vi "VIH UI - Property Page - Group Rule.vi"() -> ()   [LabVIEW 2014]
doc: "::: VI Helpeks :::\nCopyright (c) 2000-2026 Konstantin Shifershteyn. All rights reserved."
uses:
  _VIH HelpGen.llb/VIH HelpGen Typedef - Enum - Description Mode.ctl
  _VIH HelpGen.llb/VIH HelpGen Typedef - Enum - Default,Enable,Disable.ctl
  _VIH UI Controls.llb/VIH UI Control - Button - Insert HREF.ctl
  _VIH UI Controls.llb/VIH UI Control - Button - Insert Bold.ctl
  _VIH UI Controls.llb/VIH UI Control - Button - Insert Italic.ctl
  _VIH UI Controls.llb/VIH UI Control - Button - Insert Underline.ctl
  _VIH Project Manager.llb/VIH Project Tree Typedef - Tree Refnum.ctl
  VIH UI Typedef - Property Page ExtCommand.ctl
  <vilib>/Utility/miscctls.llb/LVPositionTypeDef.ctl
  <vilib>/Utility/miscctls.llb/LVPointTypeDef.ctl
  <vilib>/Utility/miscctls.llb/LVRowAndColumnUnsignedTypeDef.ctl
  <vilib>/Utility/miscctls.llb/LVSelectionTypeDef.ctl
  _VIH Support Library.llb/VIH Utility - APP - Is Value Changed (STR).vi
panel:
  out "CategoryTitle":string
  in  "%UPDATE":bool
  in  "%STOP":bool
  in  "Category List":i32(listbox)
  in  "TreeRef":T1
  in  "Tab Control":enum32{"0", "1", "2", "3", "4", "5", "6", "7"}(tab) caption="Group Rule"
  out "PI_AddInfo":string caption="Additional Information"
  out "PI_Email":string caption="Contact E-mail"
  out "PI_Website":string caption="Website"
  out "PI_Version":string caption="Version"
  out "PI_Copyright":string caption="Legal Copyright"
  out "PI_Company":string caption="Company Name"
  out "PI_Author":string caption="Author Name"
  out "PI_Product":string caption="Product Name"
  in  "ProductInfoText":string caption="Product Info section"
  in  "ProductInfoMode":u16(ring) caption="Product Info mode" items=["Default", "Custom", "Disable"]
  in  "BuildHelp":T2 caption="Build help for files of this group"
  in  "Group Name":string
  in  "Comments":string
  in  "Custom_JS Dir":i16(ring) caption="Default/Custom selector" items=["Default", "Custom"]
  in  "Dst_JS Dir":path caption="Subfolder to save JavaScript files"
  in  "Custom_CSS Dir":i16(ring) caption="Default/Custom selector" items=["Default", "Custom"]
  in  "Dst_CSS Dir":path caption="Subfolder to save CSS files"
  in  "Custom_Image Dir":i16(ring) caption="Default/Custom selector" items=["Default", "Custom"]
  in  "Dst_Image Dir":path caption="Subfolder to save image files"
  in  "Custom_HTML Dir":i16(ring) caption="Default/Custom selector" items=["Default", "Custom"]
  in  "Dst_HTML Dir":path caption="Subfolder to save HTML files"
  out "Build Root Dir":path caption="Build Root Folder"
  in  "Src_VI Template":path caption="VI Help Template File"
  in  "Custom_VI Template":i16(ring) caption="Default/Custom selector" items=["Default", "Custom"]
  in  "Src_Menu Template":path caption="Menu Help Template File"
  in  "Custom_Menu Template":i16(ring) caption="Default/Custom selector" items=["Default", "Custom"]
  in  "Src_PolyVI Template":path caption="Polymorphic VI Help Template File"
  in  "Custom_PolyVI Template":i16(ring) caption="Default/Custom selector" items=["Default", "Custom"]
  out "JS File":path caption="JS File Path"
  in  "JS List":i32[](listbox) caption="JavaScript Files"
  in  "%JS List_Add":bool caption="Add JavaScript File"
  in  "%JS List_Remove":bool caption="Remove JavaScript File"
  in  "Override_JS Files":bool caption="Override default JS file set"
  out "CSS File":path caption="CSS File Path"
  in  "CSS List":i32[](listbox) caption="CSS Files"
  in  "%CSS List_Add":bool caption="Add CSS File"
  in  "%CSS List_Remove":bool caption="Remove CSS File"
  in  "Override_CSS Files":bool caption="Override default CSS file set"
  in  "VIDetailsMode":T3 caption="Default VI details mode"
  in  "PVIIDscrMode":T3 caption="Default Polymorphic VI Instance description mode"
  in  "MenuItemIcons":T2 caption="Generate Palette Item Icons"
  in  "MenuDscrMode":T3 caption="Default Palette description mode"
  in  "VIDscrMode":T3 caption="Default VI description mode"
  in  "Ctl_EnumValues":T2 caption="Build list of Enum and Ring values"
  in  "Ctl_ClustMembers":T2 caption="Expand cluster members"
  in  "Ctl_DscrMode":T3 caption="VI Controls/Terminals description mode"
  in  "%CtrlRule_Insert_<I>":T4 caption="Format as Italic"
  in  "%CtrlRule_Insert_<U>":T5 caption="Format as Underline"
  in  "%CtrlRule_Insert_<B>":T6 caption="Format as Bold"
  in  "%CtrlRule_Insert_HREF":T7 caption="Insert Reference"
  in  "CtrlRule_Description":string caption="Description"
  in  "CtrlRule_CustomName":string caption="Custom Control Name"
  in  "CtrlRule_DscrMode":T3 caption="Description mode"
  in  "CtrlRule_CustomRule":bool caption="Enable custom rule"
  in  "CtrlRule_CtrlID":string caption="Control Identifier"
  in  "%CtrlRule_Edit_Enum":bool caption="Edit Enumerated Values Description"
  in  "CtrlRule_EnumValues":T2 caption="Enum and Ring values"
  in  "CtrlRule_ClustMembers":T2 caption="Cluster members"
  in  "%CtrlRule_Copy":bool caption="Copy"
  in  "%CtrlRule_Paste":bool caption="Paste"
  in  "%CtrlRule_Import":bool caption="Import VI Terminal Controls"
  in  "CtrlRule List":i32[](listbox) caption="Control List"
  in  "%CtrlRule_Remove":bool caption="Remove"
  in  "%CtrlRule_Add":bool caption="Add"
  in  "Override_Ctl Rules":bool caption="Override default Control Rules definition"
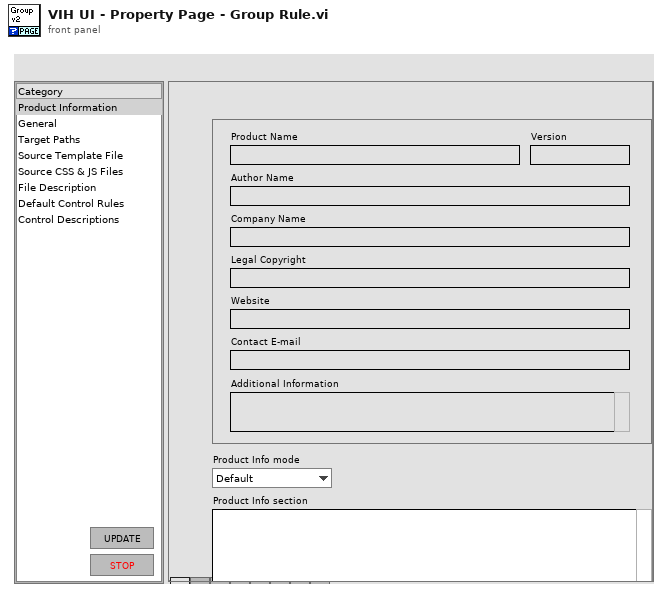
[diagram p1: front panel]
types:
  T1 = typedef "VIH Project Tree Typedef - Tree Refnum.ctl" = refnum<vi>
  T2 = typedef "VIH HelpGen Typedef - Enum - Default,Enable,Disable.ctl" = enum16{"Default", "Enable", "Disable"}
  T3 = typedef "VIH HelpGen Typedef - Enum - Description Mode.ctl" = enum16{"Default", "Description", "Description1", "Description2", "Custom", "None"}
  T4 = typedef "VIH UI Control - Button - Insert Italic.ctl" = bool
  T5 = typedef "VIH UI Control - Button - Insert Underline.ctl" = bool
  T6 = typedef "VIH UI Control - Button - Insert Bold.ctl" = bool
  T7 = typedef "VIH UI Control - Button - Insert HREF.ctl" = bool
  T8 = typedef "VIH UI Typedef - Property Page ExtCommand.ctl" = cluster{"Action":string, "Project Tree":T1, "Params":string[]}
  T9 = enum16{"Open", "Close", "Update", "Set Category"}
  T10 = enum32{"Invalid", "Standard", "Closed", "Hidden", "Minimized", "Maximized"}
  T11 = enum8{"Enabled", "Disabled", "Disabled and Grayed Out"}
  T12 = typedef "LVSelectionTypeDef.ctl" = cluster{"Selection Start":u32, "Selection End":u32}
  T13 = enum16{"get", "get all", "set", "Init", "delete"}
  T14 = typedef "eventvkey.ctl" = enum16{"ASCII", "Enter", "Return", "Shift", "Ctrl", "Alt", "Cmd", "Opt", "Caps", "NumLock", "Clear", "Break", "Up", "Down", "Left", "Right", "Insert", "Delete", "Home", "End", "PageUp", "PageDown", "Escape", "Help", "Pause", "ScrollLock", "F1", "F2", "F3", "F4", "F5", "F6", "F7", "F8", "F9", "F10", "F11", "F12", "F13", "F14", "F15", "F16", "F17", "F18", "F19", "F20", "F21", "F22", "F23", "F24", "Play", "VolumeUp", "VolumeDown", "Mute", "Two Byte Char"}
  T15 = cluster{"Shift":bool, "Ctrl":bool, "Alt":bool, "Cmd":bool, "Opt":bool}
  T16 = typedef "VIH HelpGen Typedef - Cluster - Group Rule.ctl" = cluster{"Source Root Dir":path, "Build Root Dir":path, "BuildHelp":T2, "Source Paths":T17, "Target Paths":T18, "VIDscrMode":T3, "MenuDscrMode":T3, "MenuItemIcons":T2, "Control Rules":T19[], "Flags":T21, "Ctl_DscrMode":T3, "Ctl_ClustMembers":T2, "Ctl_EnumValues":T2, "%Comments":string, "PVIIDscrMode":T3, "VIDetailsMode":T3, "ProductInfoMode":T2, "ProductInfoText":string}
  T17 = typedef "VIH HelpGen Typedef - Cluster - Group Rule - Source Paths.ctl" = cluster{"CSS Files":path[], "JS Files":path[], "VI Template":path, "Menu Template":path, "PolyVI Template":path}
  T18 = typedef "VIH HelpGen Typedef - Cluster - Group Rule - Target Paths.ctl" = cluster{"HTML Dir":path, "Image Dir":path, "CSS Dir":path, "JS Dir":path}
  T19 = typedef "VIH HelpGen Typedef - Cluster - Control Rule.ctl" = cluster{"CtrlID":string, "CustomRule":bool, "DscrMode":T3, "Description":string, "ClusterMembers":T2, "EnumValues":T2, "EnumValDscr":T20[], "CustomName":string}
  T20 = typedef "VIH HelpGen Typedef - Cluster - Enum Value Info.ctl" = cluster{"Value":ext, "String":string, "Description":string}
  T21 = typedef "VIH HelpGen Typedef - Cluster - Group Rule - Flags.ctl" = cluster{"Override CSS Files":bool, "Override JS Files":bool, "Override Ctl Rules":bool}
  T22 = typedef "LVPoint32TypeDef.ctl" = cluster{"Horizontal":i32, "Vertical":i32}
  T23 = typedef "LVRowAndColumnTypeDef.ctl" = cluster{"Row":i32, "Column":i32}
  T24 = typedef "lveventtype.ctl" = enum32{"Null", "Timeout", "Annotation Menu Selection", "Annotation Menu Selection?", "App Instance Close", "App Instance Close?", "Autoscale Range Change", "Bookmark Info Change", "Cell Edit", "Cell Edit?", "Cursor Grab", "Cursor Grab?", "Cursor Menu Selection", "Cursor Menu Selection?", "Cursor Move", "Cursor Release", "Data Change", "Direction Change", "Display State Change", "Drag Ended", "Drag Enter", "Drag Leave", "Drag Over", "Drag Source Update", "Drag Starting", "Drag Starting?", "Drop", "Exec State Change", "Key Down", "Key Down?", "Key Repeat", "Key Repeat?", "Key Up", "Listbox Double Click", "Menu Activation?", "Menu Selection (App)", "Menu Selection? (App)", "Menu Selection (User)", "Mouse Down", "Mouse Down?", "Mouse Enter", "Mouse Leave", "Mouse Move", "Mouse Up", "Mouse Wheel", "NI Security User Change (App)", "Pane Size", "Panel Close", "Panel Close?", "Panel Resize", "Plot Attribute Change", "Scale Range Change", "Shortcut Menu Activation?", "Shortcut Menu Selection (App)", "Shortcut Menu Selection? (App)", "Shortcut Menu Selection (User)", "Tree Double Click", "Tree Drag", "Tree Drag?", "Tree Drop", "Tree Drop?", "Tree Item Close", "Tree Item Close?", "Tree Item Open", "Tree Item Open?", "User Event", "Value Change"}
  T25 = typedef "LVPointTypeDef.ctl" = cluster{"Horizontal":i16, "Vertical":i16}
  T26 = typedef "LVPositionTypeDef.ctl" = cluster{"Left":i32, "Top":i32}
  T27 = typedef "LVRowAndColumnUnsignedTypeDef.ctl" = cluster{"Row":u32, "Column":u32}
  T28 = cluster{"Array out":string[], "Group Rule out":T16}
  T29 = typedef "VIH HelpGen Typedef - Product Info Cluster.ctl" = cluster{"ProductName":string, "Version":string, "Author":string, "Company":string, "Copyright":string, "Website":string, "Email":string, "AddInfo":string}
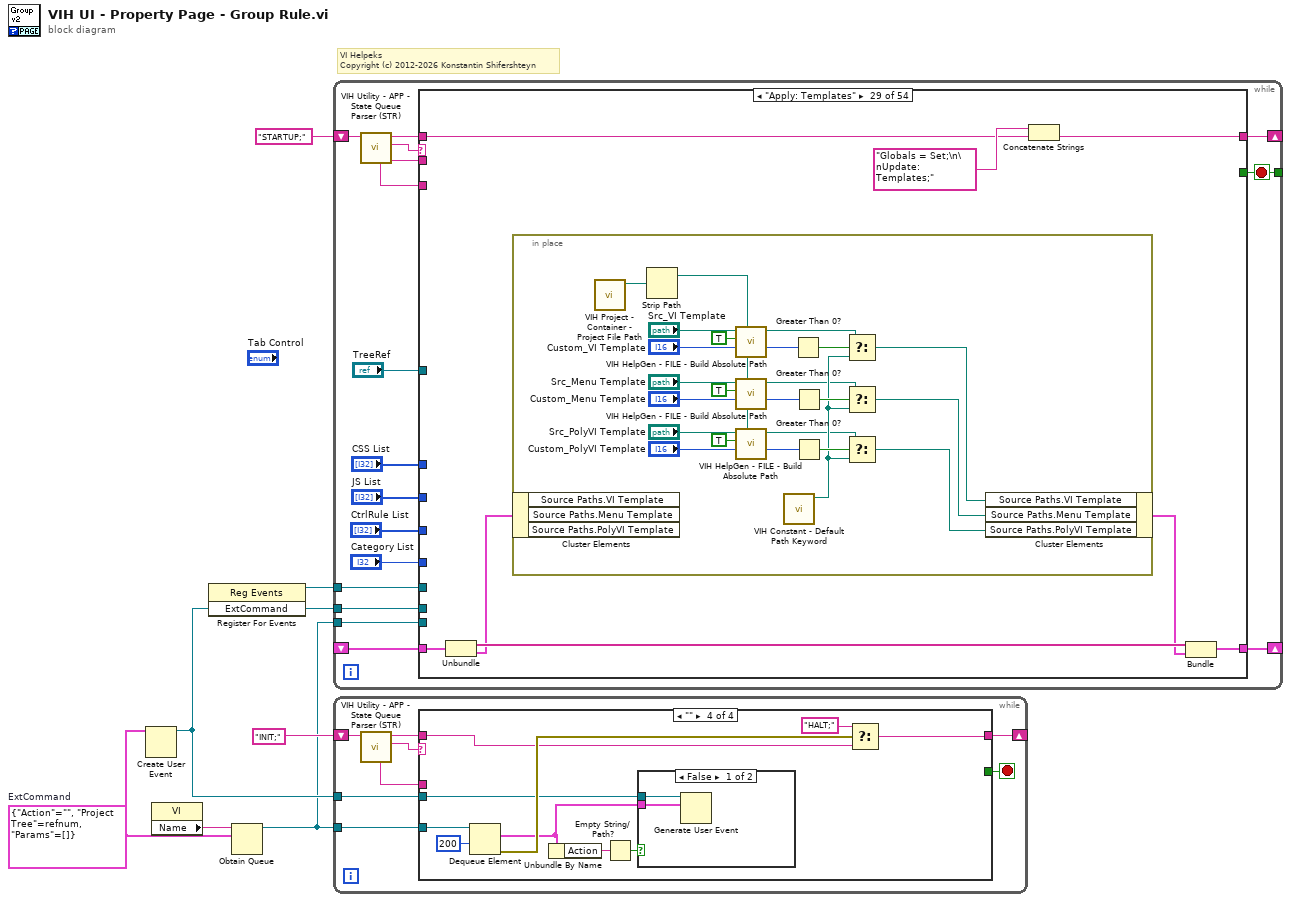
[diagram p0: block diagram]
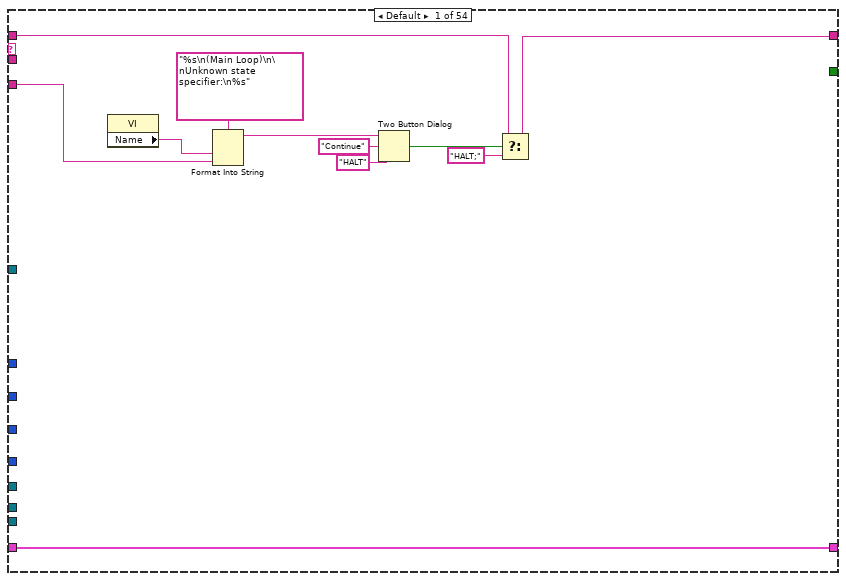
[diagram p2: hidden frame]
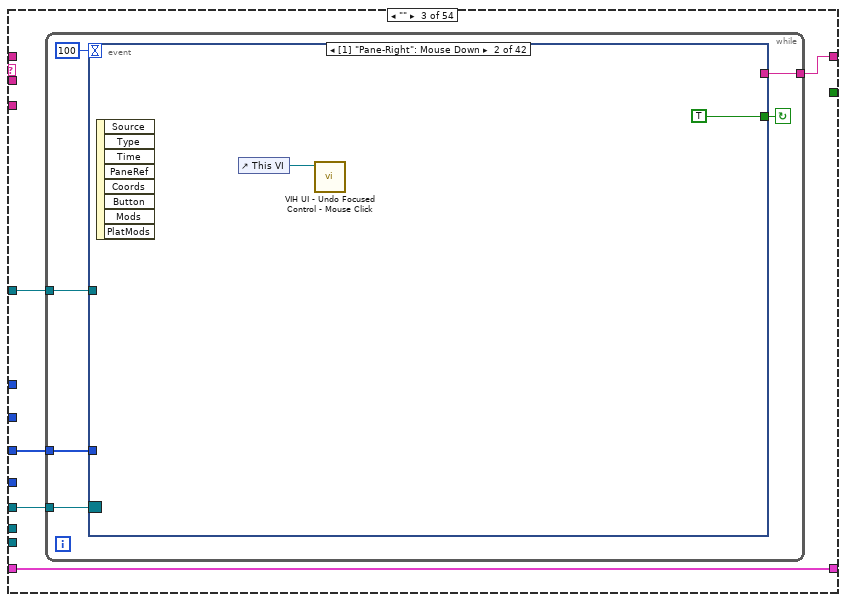
[diagram p4: hidden frame]
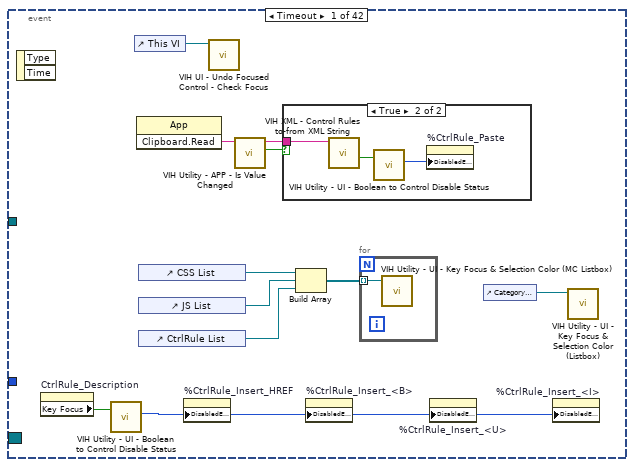
[diagram p5: hidden frame]
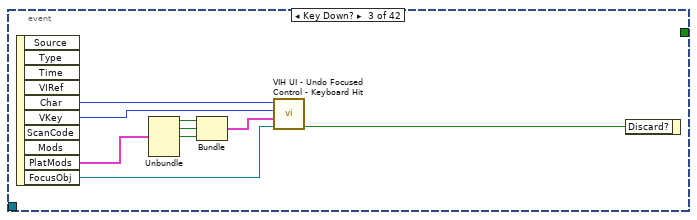
[diagram p7: hidden frame]
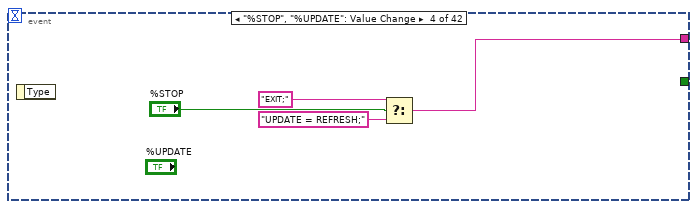
[diagram p8: hidden frame]
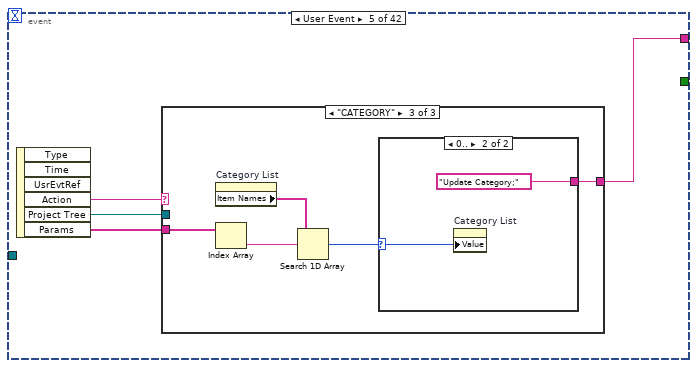
[diagram p9: hidden frame]
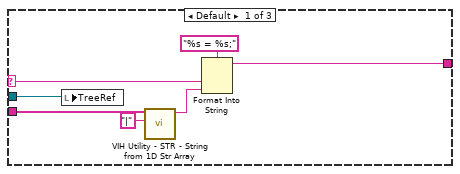
[diagram p10: hidden frame]
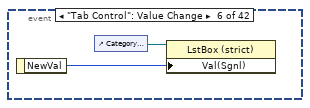
[diagram p13: hidden frame]
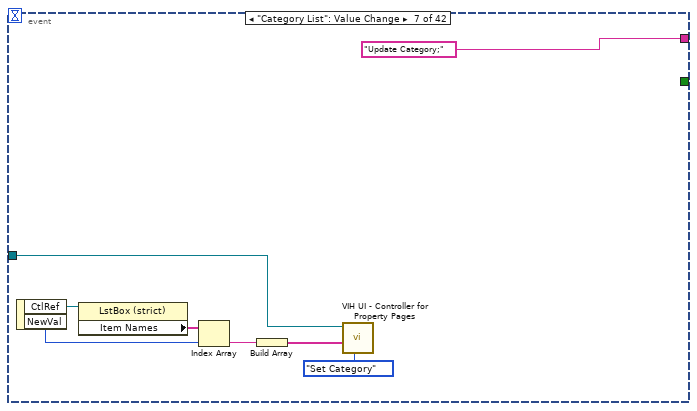
[diagram p14: hidden frame]
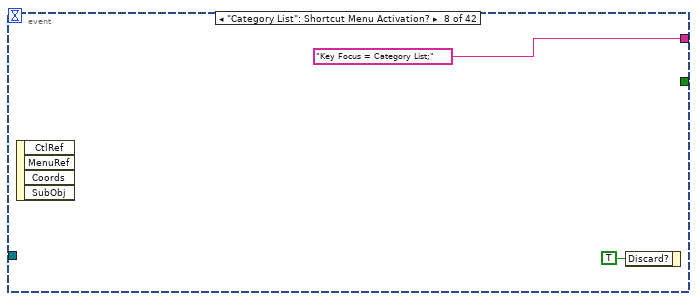
[diagram p15: hidden frame]
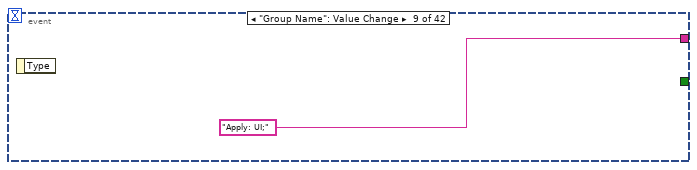
[diagram p16: hidden frame]
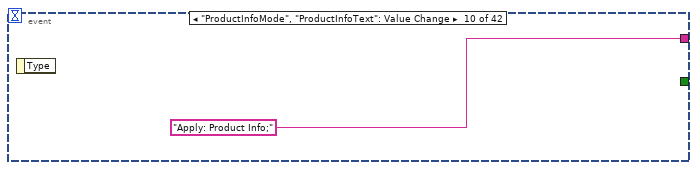
[diagram p17: hidden frame]
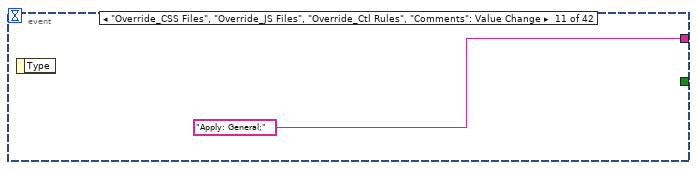
[diagram p18: hidden frame]
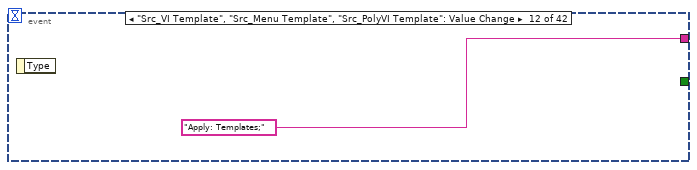
[diagram p19: hidden frame]
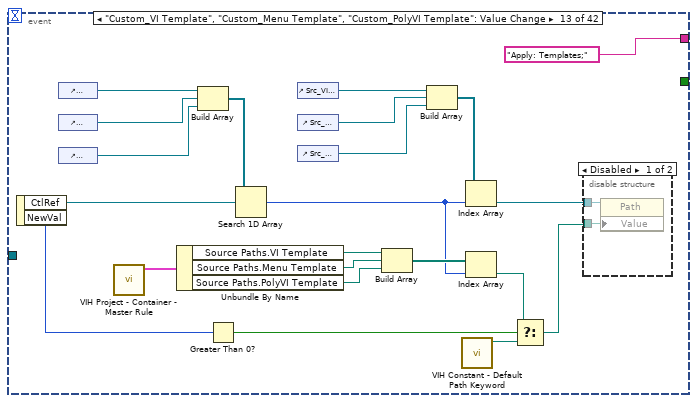
[diagram p20: hidden frame]
diagram:
  w1 = T8 {"Action"="", "Project Tree"=refnum, "Params"=[]}  # ExtCommand
  # "VI Helpeks\nCopyright (c) 2012-2026 Konstantin Shifershteyn"
  n1 = Create User Event(user event datatype=w1) -> (user event=w3:refnum<user-event>)  [unwired: 1 in, 1 out]
  n2 = property class="VI"() -> ("Name"=w6:string)  [unwired: 2 in, 2 out]
  n3 = register-events(w3) -> (reference out=w5:refnum<event-registration>)  [unwired: 2 in, 1 out]
  n4 = Obtain Queue(name (unnamed)=w6, element data type=w1) -> (queue out=w2:refnum<queue>)  [unwired: 3 in, 2 out]
  n5 = while {
    shift-right: [w21] -> _
    shift-left: "STARTUP;" -> [w24]
    tunnel: [w19] -> _
    tunnel: w5 -> [w18]
    tunnel: w3 -> [w17]
    tunnel: w2 -> [w16]
    shift-right: [w13] -> _
    shift-left: _ -> [w12]
    stop <- w19 stop-if-true
    n6 = call "VIH Utility - APP - State Queue Parser (STR).vi"("input queue"=w24) -> ("state parameters"=w15:string, "state"=w23:string, "remained queue"=w20:string, "complete state specifier"=w22:string)  [unwired: 5 in]
    n7 = case shown="\"Apply: Templates\"" w23 {
      tunnel: w22 -> [w31 _ _ _ _ _ _ _ _ w438 _ _ _ _ _ _ _ _ _ _ _ _ _ _ _ _ _ _ _ _ _ _ _ _ _ _ _ _ _ _ _ _ _ _ _ _ _ _ _ _ _ _ _ _]
      tunnel: [w26 w36 w41 "INIT;\nUPDATE;" w383 "HALT;" w411 w414 w430 w440 w463 w466 w470 w486 w493 w510 w519 w563 w602 w636 w663 w682 w697 w715 w726 w727 w740 w753 w778 w807 w824 w842 w872 w899 w948 w955 w979 w995 w1031 w1051 w1075 w1084 w1093 w1105 w1131 w1155 w1170 w1179 w1188 w1200 w1226 w1250 w1265 w1267] -> w21
      tunnel: w20 -> [w27 w36 _ _ w383 _ w411 w414 w431 w440 w463 w466 w470 w486 w493 w510 w519 w563 w602 w636 w663 w682 w697 w715 w726 w728 w746 w754 w779 w808 w824 w842 w877 w901 w948 w960 w984 w1002 w1036 w1058 w1075 w1084 w1093 w1109 w1136 w1160 w1170 w1179 w1188 w1204 w1231 w1255 w1265 w1267]
      tunnel: [_ _ _ _ _ _ TRUE _ _ _ _ _ _ _ _ _ _ _ _ _ _ _ _ _ _ _ _ _ _ _ _ _ _ _ _ _ _ _ _ _ _ _ _ _ _ _ _ _ _ _ _ _ _ _] -> w19
      tunnel: w18 -> [_ _ w42 _ _ _ w410 _ _ _ _ _ _ _ _ _ _ _ _ _ _ _ _ _ _ _ _ _ _ _ _ _ _ _ _ _ _ _ _ _ _ _ _ _ _ _ _ _ _ _ _ _ _ _]
      tunnel: w17 -> [_ _ _ _ _ _ w409 _ _ _ _ _ _ _ _ _ _ _ _ _ _ _ _ _ _ _ _ _ _ _ _ _ _ _ _ _ _ _ _ _ _ _ _ _ _ _ _ _ _ _ _ _ _ _]
      tunnel: w16 -> [_ _ _ _ _ _ w407 _ _ _ _ _ _ _ _ _ _ _ _ _ _ _ _ _ _ _ _ _ _ _ _ _ _ _ _ _ _ _ _ _ _ _ _ _ _ _ _ _ _ _ _ _ _ _]
      tunnel: w15 -> [_ _ _ _ _ _ _ _ w418 w439 _ w464 w468 _ _ _ _ _ _ w625 w654 _ w684 _ _ _ _ _ _ _ _ w825 _ w894 _ _ _ w993 w1020 w1049 _ _ _ _ _ _ _ _ _ _ _ _ _ _]
      tunnel: "Category List" -> [_ _ _ _ _ _ _ _ _ _ w460 _ _ _ _ _ _ _ _ _ _ _ _ _ _ _ _ _ _ _ _ _ _ _ _ _ _ _ _ _ _ _ _ _ _ _ _ _ _ _ _ _ _ _]
      tunnel: [w25 w37 w40 w348 w382 w392 w405 w413 w428 w442 w459 w465 w469 w485 w489 w509 w518 w562 w601 w635 w662 w681 w696 w714 w721 w732 w743 w758 w783 w812 w823 w841 w873 w898 w945 w956 w980 w997 w1032 w1053 w1074 w1081 w1092 w1106 w1132 w1156 w1169 w1176 w1187 w1201 w1227 w1251 w1264 w1266] -> w13
      tunnel: w12 -> [w25 w37 w40 w348 w382 w392 w405 w413 w425 w441 w459 w465 w469 w485 w489 w509 w518 w562 w601 w635 w662 w681 w696 w714 w721 w734 w745 w760 w785 w814 w823 w841 w874 w900 w945 w957 w981 w998 w1033 w1054 w1074 w1081 w1092 w1107 w1133 w1157 w1169 w1176 w1187 w1202 w1228 w1252 w1264 w1266]
      tunnel: "CtrlRule List" -> [_ _ w39 _ _ _ _ _ _ _ _ _ _ _ _ _ _ _ _ _ _ _ w686 _ _ _ _ _ _ _ _ w831 w866 w892 w946 w953 _ _ _ _ _ _ _ _ _ _ _ _ _ _ _ _ _ _]
      tunnel: "CSS List" -> [_ _ _ _ _ _ _ _ _ _ _ _ _ _ _ _ _ _ _ w627 _ _ _ _ _ _ _ _ _ _ _ _ _ _ _ _ _ _ _ _ _ w1078 _ w1097 w1129 _ _ _ _ _ _ _ _ _]
      tunnel: "JS List" -> [_ _ _ _ _ _ _ _ _ _ _ _ _ _ _ _ _ _ _ _ w653 _ _ _ _ _ _ _ _ _ _ _ _ _ _ _ _ _ _ _ _ _ _ _ _ _ _ w1171 _ w1190 w1224 _ _ _]
      tunnel: "TreeRef" -> [_ _ w38 _ _ _ _ _ _ _ _ _ _ _ w490 _ _ w535 w578 _ _ _ _ _ w719 _ _ _ _ _ _ _ _ w890 _ _ _ _ _ w1048 _ _ _ _ _ _ _ _ _ _ _ _ _ _]
      frame Default {
        n8 = property class="VI"() -> ("Name"=w30:string)  [unwired: 2 in, 2 out]
        n9 = Format Into String(format string="%s\n(Main Loop)\n\nUnknown state specifier:\n%s", w30, w31) -> (resulting string=w34:string)  [unwired: 2 in, 1 out]
        n10 = Two Button Dialog(message=w34, 1:"HALT" ("F button name (\"Cancel\")"), 2:"Continue" ("T button name (\"OK\")")) -> (T button?=w28:bool)
        n11 = Select(t=w27, s=w28, f="HALT;") -> (s? t:f=w26:string)
      }
      frame "#" {
      }
      frame "" {
        n12 = while {
          tunnel: w42 -> [w47]
          tunnel: [w46] -> w41
          tunnel: w39 -> [w45]
          tunnel: w38 -> [w44]
          stop <- w43 continue-if-true
          n13 = event shown="[1] \"Pane-Right\": Mouse Down" {
            selector: w47 -> [_ _ _ _ _ _ _ _ _ _ _ _ _ _ _ _ _ _ _ _ _ _ _ _ _ _ _ _ _ _ _ _ _ _ _ _ _ _ _ _ _ _]
            dyn-events: _ -> [_ _ _ _ _ _ _ _ _ _ _ _ _ _ _ _ _ _ _ _ _ _ _ _ _ _ _ _ _ _ _ _ _ _ _ _ _ _ _ _ _ _]
            timeout: 100 -> [_ _ _ _ _ _ _ _ _ _ _ _ _ _ _ _ _ _ _ _ _ _ _ _ _ _ _ _ _ _ _ _ _ _ _ _ _ _ _ _ _ _]
            tunnel: [_ _ _ w76 w82 _ "Update Category;" ("string") "Key Focus = Category List;" ("output string") "Apply: UI;" ("string") "Apply: Product Info;" ("string") "Apply: General;" ("string") "Apply: Templates;" ("string") "Apply: Templates;" ("string") "Apply: Target Paths;" ("string") "Apply: Target Paths;" ("string") "Apply: Item Rules;" ("string") "Apply: Item Rules;" ("string") "CtrlRule: Update Controls = INIT;" ("string") w181 w195 w210 w225 "Key Focus = CtrlRule List;" ("output string") w229 w239 w252 w258 "CSS List: Update Controls;" w264 "Key Focus = CSS List;" ("output string") w268 "JS List: Update Controls;" w277 "Key Focus = JS List;" ("output string") w281 _ _ _ _ _ _ _] -> w46
            tunnel: w45 -> [_ _ _ _ _ _ _ _ _ _ _ _ _ _ _ _ _ _ _ w193 _ _ _ _ _ w245 w255 _ _ _ _ _ _ _ _ _ _ _ _ _ _ _]
            tunnel: w44 -> [_ _ _ _ _ _ w99 _ _ _ _ _ _ _ _ _ _ _ _ _ _ _ _ _ _ _ _ _ _ _ _ _ _ _ _ w293 w301 w307 w310 w316 w319 w325]
            tunnel: [_ TRUE _ _ _ _ _ _ _ _ _ _ _ _ _ _ _ _ _ _ _ _ _ _ _ _ _ _ _ _ _ _ _ _ _ _ _ _ _ _ _ _] -> w43
            event Timeout {
              n14 = event-data() -> ()  [unwired: 1 in, 2 out]
              n15 = property on="CtrlRule_Description" class="Str"() -> ("Key Focus"=w51:bool)  [unwired: 2 in, 2 out]
              n16 = call "VIH Utility - UI - Boolean to Control Disable Status.vi"("Status in"=w51) -> ("Control Disable if False"=w50:u8)  [unwired: 3 in, 1 out]
              n17 = control-ref of="This VI"() -> (w49:refnum<vi>)
              n18 = invoke class="App" method="Clipboard.Read"() -> ("Read Clipbrd"=w54:string)  [unwired: 3 in, 2 out]
              n19 = control-ref of="CSS List"() -> (w57:refnum<vi>)
              n20 = control-ref of="JS List"() -> (w56:refnum<vi>)
              n21 = control-ref of="CtrlRule List"() -> (w55:refnum<vi>)
              n22 = property on="%CtrlRule_Insert_HREF" class="Bool"("DisabledEnum"=w50) -> ()  [unwired: 2 in, 2 out]
              n23 = call "VIH UI - Undo Focused Control - Check Focus.vi"("VI Refnum"=w49) -> ()  [unwired: 10 in, 1 out]
              n24 = call-poly "VIH Utility - APP - Is Value Changed.vi"("Value"=w54) -> ("Changed"=w52:bool, "dup Value"=w53:string)  [unwired: 5 in]
              n25 = case shown="True" w52 {
                tunnel: w53 -> [_ w60]
                frame False {
                }
                frame True {
                  n26 = call "VIH XML - Control Rules to-from XML String.vi"("XML in"=w60) -> ("available"=w62:bool)  [unwired: 7 in, 3 out]
                  n27 = call "VIH Utility - UI - Boolean to Control Disable Status.vi"("Status in"=w62) -> ("Control Disable if False"=w61:u8)  [unwired: 3 in, 1 out]
                  n28 = property on="%CtrlRule_Paste" class="Bool"("DisabledEnum"=w61) -> ()  [unwired: 2 in, 2 out]
                }
              }
              n29 = Build Array(w57, w56, w55) -> (w59:refnum<vi>[])
              n30 = property on="%CtrlRule_Insert_<B>" class="Bool"("DisabledEnum"=w50) -> ()  [unwired: 2 in, 2 out]
              n31 = for {
                tunnel: w59 -> [w63] mode=indexing
                n32 = call "VIH Utility - UI - Key Focus & Selection Color (MC Listbox).vi"("MCListbox Refnum"=w63) -> ()  [unwired: 8 in, 3 out]
              }
              n33 = property on="%CtrlRule_Insert_<U>" class="Bool"("DisabledEnum"=w50) -> ()  [unwired: 2 in, 2 out]
              n34 = control-ref of="Category List"() -> (w58:refnum<vi>)
              n35 = property on="%CtrlRule_Insert_<I>" class="Bool"("DisabledEnum"=w50) -> ()  [unwired: 2 in, 2 out]
              n36 = call "VIH Utility - UI - Key Focus & Selection Color (Listbox).vi"("LstBox Refnum"=w58) -> ()  [unwired: 8 in, 3 out]
            }
            event Mouse Down {
              n37 = event-data() -> ()  [unwired: 1 in, 8 out]
              n38 = control-ref of="This VI"() -> (w65:refnum<vi>)
              n39 = call "VIH UI - Undo Focused Control - Mouse Click.vi"("VI Refnum"=w65) -> ()  [unwired: 9 in, 2 out]
            }
            event Key Down? {
              n40 = event-data() -> ("Char"=w70:i16, "VKey"=w69:T14, "PlatMods"=w68:T15, "FocusObj"=w67:refnum<vi>)  [unwired: 1 in, 6 out]
              n41 = Unbundle(w68) -> ("Shift"=w71:bool, "Ctrl"=w72:bool, "Alt"=w73:bool)  [unwired: 2 out]
              n42 = Bundle("Shift"=w71, "Ctrl"=w72, "Alt"=w73) -> (w74:cluster{"Shift":bool, "Ctrl":bool, "Alt":bool})  [unwired: 1 in]
              n43 = call "VIH UI - Undo Focused Control - Keyboard Hit.vi"("FocusObj"=w67, "PlatMods"=w74, "VKey"=w69, "Char"=w70) -> ("Discard"=w66:bool)  [unwired: 7 in]
              n44 = event-data("Discard?"=w66) -> ()  [unwired: 1 in, 1 out]
            }
            event "%STOP", "%UPDATE": Value Change {
              n45 = event-data() -> ()  [unwired: 1 in, 1 out]
              n46 = Select(t="EXIT;", s="%STOP", f="UPDATE = REFRESH;") -> (s? t:f=w76:string)
            }
            event User Event {
              n47 = event-data() -> ("Action"=w80:string, "Project Tree"=w79:T1, "Params"=w81:string[])  [unwired: 1 in, 3 out]
              n48 = case shown="\"CATEGORY\"" w80 {
                selector: w80 -> [w84 _ _]
                tunnel: w81 -> [w89 _ w94]
                tunnel: [w85 _ w90] -> w82
                tunnel: w79 -> [w83 _ _]
                frame Default {
                  n49 = local write "TreeRef"(w83) -> ()
                  n50 = call "VIH Utility - STR - String from 1D Str Array.vi"("delimiter ('\\n')"="|" ("delimiter ('\\n')"), "Array in"=w89) -> ("String out"=w86:string)  [unwired: 5 in]
                  n51 = Format Into String(format string="%s = %s;", w84, w86) -> (resulting string=w85:string)  [unwired: 2 in, 1 out]
                }
                frame "" {
                }
                frame "CATEGORY" {
                  n52 = property on="Category List" class="LstBox (strict)"() -> ("Item Names"=w92:string[])  [unwired: 2 in, 2 out]
                  n53 = Index Array(array=w94) -> (element=w93:string)  [unwired: 1 in]
                  n54 = Search 1D Array(1D array=w92, element=w93) -> (index of element=w91:i32)  [unwired: 1 in]
                  n55 = case shown="0.." w91 {
                    selector: w91 -> [_ w96]
                    tunnel: [_ "Update Category;" ("string")] -> w90
                    frame ..-1 {
                    }
                    frame 0.. {
                      n56 = property on="Category List" class="LstBox (strict)"("Value"=w96) -> ()  [unwired: 2 in, 2 out]
                    }
                  }
                }
              }
            }
            event "Tab Control": Value Change {
              n57 = event-data() -> ("NewVal"=w98:enum32{"0", "1", "2", "3", "4", "5", "6", "7"})  [unwired: 1 in]
              n58 = control-ref of="Category List"() -> (w97:refnum<vi>)
              n59 = property class="LstBox (strict)"(reference=w97, "Val(Sgnl)"=w98) -> ()  [unwired: 1 in, 2 out]
            }
            event "Category List": Value Change {
              n60 = event-data() -> ("CtlRef"=w105:refnum<vi>, "NewVal"=w103:i32)  [unwired: 1 in]
              n61 = property class="LstBox (strict)"(reference=w105) -> ("Item Names"=w104:string[])  [unwired: 1 in, 2 out]
              n62 = Index Array(array=w104, index=w103) -> (element=w100:string)
              n63 = Build Array(w100) -> (w101:string[])
              n64 = call "VIH UI - Controller for Property Pages.vi"("cmd (update)"=T9."Set Category", "Params"=w101, "Project Tree"=w99) -> ()  [unwired: 7 in, 2 out]
            }
            event "Category List": Shortcut Menu Activation? {
              n65 = event-data() -> ()  [unwired: 1 in, 4 out]
              n66 = event-data("Discard?"=TRUE) -> ()  [unwired: 1 in, 1 out]
            }
            event "Group Name": Value Change {
              n67 = event-data() -> ()  [unwired: 1 in, 1 out]
            }
            event "ProductInfoMode", "ProductInfoText": Value Change {
              n68 = event-data() -> ()  [unwired: 1 in, 1 out]
            }
            event "Override_CSS Files", "Override_JS Files", "Override_Ctl Rules", "Comments": Value Change {
              n69 = event-data() -> ()  [unwired: 1 in, 1 out]
            }
            event "Src_VI Template", "Src_Menu Template", "Src_PolyVI Template": Value Change {
              n70 = event-data() -> ()  [unwired: 1 in, 1 out]
            }
            event "Custom_VI Template", "Custom_Menu Template", "Custom_PolyVI Template": Value Change {
              n71 = event-data() -> ("CtlRef"=w119:refnum<vi>, "NewVal"=w128:i16)  [unwired: 1 in]
              n72 = control-ref of="Custom_VI Template"() -> (w126:refnum<vi>)
              n73 = control-ref of="Custom_Menu Template"() -> (w125:refnum<vi>)
              n74 = control-ref of="Custom_PolyVI Template"() -> (w114:refnum<vi>)
              n75 = call "VIH Project - Container - Master Rule.vi"() -> ("Rule out"=w124:T16)  [unwired: 11 in]
              n76 = Unbundle By Name(w124) -> ("Source Paths.VI Template"=w123:path, "Source Paths.Menu Template"=w122:path, "Source Paths.PolyVI Template"=w115:path)
              n77 = Build Array(w126, w125, w114) -> (w133:refnum<vi>[])
              n78 = Greater Than 0?(x=w128) -> (x > 0?=w118:bool)
              n79 = Search 1D Array(1D array=w133, element=w119) -> (index of element=w117:i32)  [unwired: 1 in]
              n80 = control-ref of="Src_VI Template"() -> (w132:refnum<vi>)
              n81 = control-ref of="Src_Menu Template"() -> (w131:refnum<vi>)
              n82 = control-ref of="Src_PolyVI Template"() -> (w113:refnum<vi>)
              n83 = Build Array(w123, w122, w115) -> (w121:path[])
              n84 = Build Array(w132, w131, w113) -> (w130:refnum<vi>[])
              n85 = call "VIH Constant - Default Path Keyword.vi"() -> ("<default> path"=w116:path)  [unwired: 11 in]
              n86 = Index Array(array=w130, index=w117) -> (element=w129:refnum<vi>)
              n87 = Index Array(array=w121, index=w117) -> (element=w120:path)
              n88 = Select(t=w120, s=w118, f=w116) -> (s? t:f=w127:path)
              n89 = disable-structure shown="Disabled" {
                disable-tunnel: w129 -> [w136 _]
                disable-tunnel: w127 -> [w135 _]
                frame Disabled {
                  n90 = property class="Path"(reference=w136, "Value"=w135) -> ()  [unwired: 1 in, 2 out]
                }
                frame Enabled {
                }
              }
            }
            event "Dst_HTML Dir", "Dst_Image Dir", "Dst_CSS Dir", "Dst_JS Dir": Value Change {
              n91 = event-data() -> ("CtlRef"=w139:refnum<vi>, "NewVal"=w137:path)  [unwired: 1 in]
              n92 = Empty String/Path?(string/path=w137) -> (empty?=w138:bool)
              n93 = case shown="False" w138 {
                tunnel: w139 -> [w143 _]
                tunnel: w137 -> [w141 _]
                frame False {
                  n94 = Path Type(1:w141) -> (0:w142:i16)
                  n95 = case shown="0" w142 {
                    tunnel: w143 -> [w148 _ w150]
                    tunnel: w141 -> [w145 _ _]
                    frame 0 {
                      # "If absolute path was enered"
                      n96 = call "VIH Project - Container - Master Rule.vi"() -> ("Rule out"=w147:T16)  [unwired: 11 in]
                      n97 = Unbundle By Name(w147) -> ("Build Root Dir"=w144:path)
                      n98 = call "VIH HelpGen - FILE - Build Relative Path.vi"("Root Path"=w144, "Path in"=w145) -> ("Path out"=w146:path)  [unwired: 9 in]
                      n99 = property class="Path"(reference=w148, "Value"=w146) -> ()  [unwired: 1 in, 2 out]
                    }
                    frame 1 {
                    }
                    frame 2, Default {
                      # "Not A Path"
                      n100 = property class="Path"(reference=w150, "Value"=path "") -> ()  [unwired: 1 in, 2 out]
                    }
                  }
                }
                frame True {
                }
              }
            }
            event "Custom_HTML Dir", "Custom_Image Dir", "Custom_CSS Dir", "Custom_JS Dir": Value Change {
              n101 = event-data() -> ("CtlRef"=w153:refnum<vi>, "NewVal"=w163:i16)  [unwired: 1 in, 1 out]
              n102 = control-ref of="Custom_HTML Dir"() -> (w174:refnum<vi>)
              n103 = control-ref of="Custom_Image Dir"() -> (w173:refnum<vi>)
              n104 = control-ref of="Custom_CSS Dir"() -> (w172:refnum<vi>)
              n105 = control-ref of="Custom_JS Dir"() -> (w171:refnum<vi>)
              n106 = call "VIH Project - Container - Master Rule.vi"() -> ("Rule out"=w161:T16)  [unwired: 11 in]
              n107 = Build Array(w174, w173, w172, w171) -> (w170:refnum<vi>[])
              n108 = Unbundle By Name(w161) -> ("Target Paths.HTML Dir"=w160:path, "Target Paths.Image Dir"=w159:path, "Target Paths.CSS Dir"=w158:path, "Target Paths.JS Dir"=w157:path)
              n109 = Greater Than 0?(x=w163) -> (x > 0?=w152:bool)
              n110 = Search 1D Array(1D array=w170, element=w153) -> (index of element=w155:i32)  [unwired: 1 in]
              n111 = control-ref of="Dst_HTML Dir"() -> (w169:refnum<vi>)
              n112 = control-ref of="Dst_Image Dir"() -> (w168:refnum<vi>)
              n113 = control-ref of="Dst_CSS Dir"() -> (w167:refnum<vi>)
              n114 = control-ref of="Dst_JS Dir"() -> (w166:refnum<vi>)
              n115 = Build Array(w160, w159, w158, w157) -> (w156:path[])
              n116 = Build Array(w169, w168, w167, w166) -> (w165:refnum<vi>[])
              n117 = Index Array(array=w156, index=w155) -> (element=w154:path)
              n118 = Index Array(array=w165, index=w155) -> (element=w164:refnum<vi>)
              n119 = call "VIH Constant - Default Path Keyword.vi"() -> ("<default> path"=w151:path)  [unwired: 11 in]
              n120 = Select(t=w154, s=w152, f=w151) -> (s? t:f=w162:path)
              n121 = disable-structure shown="Disabled" {
                disable-tunnel: w164 -> [w177 _]
                disable-tunnel: w162 -> [w176 _]
                frame Disabled {
                  n122 = property class="Path"(reference=w177, "Value"=w176) -> ()  [unwired: 1 in, 2 out]
                }
                frame Enabled {
                }
              }
            }
            event Value Change {
              n123 = event-data() -> ()  [unwired: 1 in, 1 out]
            }
            event Value Change {
              n124 = event-data() -> ()  [unwired: 1 in, 1 out]
            }
            event "CtrlRule List": Value Change {
              n125 = event-data() -> ()  [unwired: 1 in, 1 out]
            }
            event "CtrlRule List": Double Click {
              n126 = event-data() -> ("CtlRef"=w182:refnum<vi>, "Row"=w183:i32)  [unwired: 1 in, 6 out]
              n127 = property class="MCListbox (strict)"(reference=w182) -> ("ItemNames"=w184:string[][])  [unwired: 1 in, 2 out]
              n128 = Index Array(array=w184, index (row)=w183, index (col)=1 ("disabled index (col)")) -> (element=w186:string)
              n129 = Empty String/Path?(string/path=w186) -> (empty?=w187:bool)
              n130 = case shown="False" w187 {
                tunnel: [w190 _] -> w181
                tunnel: w183 -> [w188 _]
                frame False {
                  n131 = Format Into String(format string="CtrlRule: Edit Enum Values = %d;" ("string"), w188) -> (resulting string=w190:string)  [unwired: 2 in, 1 out]
                }
                frame True {
                }
              }
            }
            event "CtrlRule List": Edit Cell {
              n132 = event-data() -> ("String"=w192:string)  [unwired: 1 in, 4 out]
              n133 = local write "CtrlRule_CtrlID"(w192) -> ()
              n134 = Index Array(array=w193) -> (element=w191:i32)  [unwired: 1 in]
              n135 = Format Into String(format string="CtrlRule: Apply = %d;" ("string"), w191) -> (resulting string=w195:string)  [unwired: 2 in, 1 out]
            }
            event "CtrlRule List": Mouse Up {
              n136 = event-data() -> ("CtlRef"=w207:refnum<vi>, "Coords"=w209:T22, "Button"=w208:u16)  [unwired: 1 in, 2 out]
              n137 = property class="MCListbox (strict)"(reference=w207) -> ("ItemSyms"=w197:i32[])  [unwired: 1 in, 2 out]
              n138 = invoke class="MCListbox (strict)" method="Point To Row Column"(reference=w207, "Point"=w209) -> ("CellPosition"=w205:T23, "InGlyph"=w200:bool)  [unwired: 5 in, 5 out]
              n139 = Equal?(x=w208, y=u16 1) -> (x = y?=w201:bool)
              n140 = Array Size(array=w197) -> (size(s)=w204:i32)
              n141 = Unbundle By Name(w205) -> ("Row"=w203:i32)
              n142 = In Range and Coerce(upper limit=w204, x=w203, lower limit=0) -> (coerced(x)=w196:i32, In Range?=w199:bool)
              n143 = Compound Arithmetic op=AND(w200, w201, w199) -> (w198:bool)
              n144 = case shown="True" w198 {
                tunnel: [_ w213] -> w210
                tunnel: w197 -> [_ w223]
                tunnel: w196 -> [_ w212]
                frame False {
                }
                frame True {
                  n145 = Index Array(array=w223, index=w212) -> (element=w221:i32)
                  n146 = Build Array(w212) -> (w217:i32[])
                  n147 = And(x=65535, y=w221) -> (x .and. y?=w220:i32)
                  n148 = Number To Decimal String(number=w217) -> (decimal integer string=w218:string[])  [unwired: 1 in]
                  n149 = Equal?(x=w220, y=37) -> (x = y?=w211:bool)
                  n150 = call "VIH Utility - STR - String from 1D Str Array.vi"("delimiter ('\\n')"="," ("delimiter ('\\n')"), "Array in"=w218) -> ("String out"=w216:string)  [unwired: 5 in]
                  n151 = Format Into String(format string="CtrlRule: Enable = %d ? %s;" ("string"), w211, w216) -> (resulting string=w213:string)  [unwired: 2 in, 1 out]
                }
              }
            }
            event "CtrlRule List": Drag Ended {
              n152 = event-data() -> ("Result"=w224:enum16{"Drop Cancel", "Drop Move", "Drop Copy"})  [unwired: 1 in, 1 out]
              n153 = case shown="\"Drop Move\"" w224 {
                tunnel: [_ "CtrlRule: Dragged;"] -> w225
                frame Default {
                }
                frame "Drop Move" {
                }
              }
            }
            event "CtrlRule List": Shortcut Menu Activation? {
              n154 = event-data() -> ()  [unwired: 1 in, 4 out]
              n155 = event-data("Discard?"=TRUE) -> ()  [unwired: 1 in, 1 out]
            }
            event "%CtrlRule_Add", "%CtrlRule_Remove": Value Change {
              n156 = event-data() -> ()  [unwired: 1 in, 1 out]
              n157 = Build Array("%CtrlRule_Add", "%CtrlRule_Remove") -> (w233:bool[])
              n158 = Search 1D Array(1D array=w233, element=TRUE) -> (index of element=w231:i32)  [unwired: 1 in]
              n159 = Pick Line(multi-line string="CtrlRule: Add;              Key Focus = CtrlRule Control ID;\nCtrlRule: Remove;       Key Focus = CtrlRule List;" ("string"), line index=w231) -> (output string=w229:string)  [unwired: 1 in]
            }
            event "%CtrlRule_Import", "%CtrlRule_Paste", "%CtrlRule_Copy": Value Change {
              n160 = event-data() -> ()  [unwired: 1 in, 1 out]
              n161 = Build Array("%CtrlRule_Import", "%CtrlRule_Paste", "%CtrlRule_Copy") -> (w243:bool[])
              n162 = Search 1D Array(1D array=w243, element=TRUE) -> (index of element=w241:i32)  [unwired: 1 in]
              n163 = Pick Line(multi-line string="CtrlRule: Import = VI;    Key Focus = CtrlRule List;\nCtrlRule: Import = CB;   Key Focus = CtrlRule List;\nCtrlRule: Export = CB;   Key Focus = CtrlRule List;" ("string"), line index=w241) -> (output string=w239:string)  [unwired: 1 in]
            }
            event "CtrlRule_CtrlID", "CtrlRule_CustomRule", "CtrlRule_Description", "CtrlRule_CustomName": Value Change {
              n164 = event-data() -> ()  [unwired: 1 in, 1 out]
              n165 = Index Array(array=w245) -> (element=w247:i32)  [unwired: 1 in]
              n166 = Array Size(array=w245) -> (size(s)=w250:i32)
              n167 = Equal?(x=w250, y=1) -> (x = y?=w248:bool)
              n168 = Select(t=w247, s=w248, f=-1) -> (s? t:f=w244:i32)
              n169 = Format Into String(format string="CtrlRule: Apply = %d;" ("string"), w244) -> (resulting string=w252:string)  [unwired: 2 in, 1 out]
            }
            event "%CtrlRule_Edit_Enum": Value Change {
              n170 = event-data() -> ()  [unwired: 1 in, 1 out]
              n171 = Index Array(array=w255) -> (element=w254:i32)  [unwired: 1 in]
              n172 = Array Size(array=w255) -> (size(s)=w257:i32)
              n173 = Equal?(x=w257, y=1) -> (x = y?=w253:bool)
              n174 = case shown="True" w253 {
                tunnel: [_ w261] -> w258
                tunnel: w254 -> [_ w259]
                frame False {
                }
                frame True {
                  n175 = Format Into String(format string="CtrlRule: Edit Enum Values = %d;" ("string"), w259) -> (resulting string=w261:string)  [unwired: 2 in, 1 out]
                }
              }
            }
            event "CSS List": Value Change {
              n176 = event-data() -> ()  [unwired: 1 in, 1 out]
            }
            event "CSS List": Drag Ended {
              n177 = event-data() -> ("Result"=w263:enum16{"Drop Cancel", "Drop Move", "Drop Copy"})  [unwired: 1 in, 1 out]
              n178 = case shown="\"Drop Move\"" w263 {
                tunnel: [_ "CSS List: Dragged;"] -> w264
                frame Default {
                }
                frame "Drop Move" {
                }
              }
            }
            event "CSS List": Shortcut Menu Activation? {
              n179 = event-data() -> ()  [unwired: 1 in, 4 out]
              n180 = event-data("Discard?"=TRUE) -> ()  [unwired: 1 in, 1 out]
            }
            event "%CSS List_Add", "%CSS List_Remove": Value Change {
              n181 = event-data() -> ()  [unwired: 1 in, 1 out]
              n182 = Build Array("%CSS List_Add", "%CSS List_Remove") -> (w274:bool[])
              n183 = Search 1D Array(1D array=w274, element=TRUE) -> (index of element=w272:i32)  [unwired: 1 in]
              n184 = Pick Line(multi-line string="CSS List: Add;         Key Focus = CSS List;\nCSS List: Remove;  Key Focus = CSS List;", line index=w272) -> (output string=w268:string)  [unwired: 1 in]
            }
            event "JS List": Value Change {
              n185 = event-data() -> ()  [unwired: 1 in, 1 out]
            }
            event "JS List": Drag Ended {
              n186 = event-data() -> ("Result"=w276:enum16{"Drop Cancel", "Drop Move", "Drop Copy"})  [unwired: 1 in, 1 out]
              n187 = case shown="\"Drop Move\"" w276 {
                tunnel: [_ "JS List: Dragged;"] -> w277
                frame Default {
                }
                frame "Drop Move" {
                }
              }
            }
            event "JS List": Shortcut Menu Activation? {
              n188 = event-data() -> ()  [unwired: 1 in, 4 out]
              n189 = event-data("Discard?"=TRUE) -> ()  [unwired: 1 in, 1 out]
            }
            event "%JS List_Add", "%JS List_Remove": Value Change {
              n190 = event-data() -> ()  [unwired: 1 in, 1 out]
              n191 = Build Array("%JS List_Add", "%JS List_Remove") -> (w287:bool[])
              n192 = Search 1D Array(1D array=w287, element=TRUE) -> (index of element=w285:i32)  [unwired: 1 in]
              n193 = Pick Line(multi-line string="JS List: Add;         Key Focus = JS List;\nJS List: Remove;  Key Focus = JS List;", line index=w285) -> (output string=w281:string)  [unwired: 1 in]
            }
            event Value Change {
              n194 = event-data() -> ()  [unwired: 1 in, 5 out]
              n195 = control-ref of="CtrlRule_Description"() -> (w294:refnum<vi>)
              n196 = Build Array("%CtrlRule_Insert_HREF", "%CtrlRule_Insert_<B>", "%CtrlRule_Insert_<I>", "%CtrlRule_Insert_<U>") -> (w295:T5[])
              n197 = Search 1D Array(1D array=w295, element=TRUE) -> (index of element=w297:i32)  [unwired: 1 in]
              n198 = Increment(x=w297) -> (x+1=w298:i32)
              n199 = Type Cast(type=enum32{"nop", "<a>", "<b>", "<i>", "<u>"}."nop" ("cmd"), x=w298) -> (*(type *) &x=w300:enum32{"nop", "<a>", "<b>", "<i>", "<u>"})
              n200 = call "VIH UI - Insert HTML Tag to String.vi"("cmd"=w300, "Project Tree"=w293, "Str Refnum"=w294) -> ("dup Str Refnum"=w288:refnum<vi>)  [unwired: 8 in]
              n201 = call "VIH UI - Undo Focused Control - Core.vi"("Ctl Refnum"=w288) -> ()  [unwired: 8 in, 3 out]
            }
            event "ProductInfoText": Shortcut Menu Activation? {
              n202 = event-data() -> ("Type"=w304:T24, "CtlRef"=w303:refnum<vi>, "MenuRef"=w302:refnum<k9>)  [unwired: 1 in, 1 out]
              n203 = call "VIH UI - String Shortcut Menu Handler.vi"("Project Tree"=w301, "mode"=enum16{"basic", "format 1", "format 2"}."format 2", "menu"=w302, "Str Refnum"=w303, "Type"=w304) -> ()  [unwired: 7 in]
              n204 = event-data() -> ()  [unwired: 2 in, 1 out]
            }
            event "ProductInfoText": Shortcut Menu Selection (User) {
              n205 = event-data() -> ("Type"=w309:T24, "CtlRef"=w308:refnum<vi>, "ItemTag"=w306:string)  [unwired: 1 in, 1 out]
              n206 = call "VIH UI - String Shortcut Menu Handler.vi"("Project Tree"=w307, "Menu tag"=w306, "Str Refnum"=w308, "Type"=w309) -> ()  [unwired: 8 in]
            }
            event "CtrlRule_Description": Shortcut Menu Activation? {
              n207 = event-data() -> ("Type"=w313:T24, "CtlRef"=w312:refnum<vi>, "MenuRef"=w311:refnum<k9>)  [unwired: 1 in, 1 out]
              n208 = call "VIH UI - String Shortcut Menu Handler.vi"("Project Tree"=w310, "mode"=enum16{"basic", "format 1", "format 2"}."format 1", "menu"=w311, "Str Refnum"=w312, "Type"=w313) -> ()  [unwired: 7 in]
              n209 = event-data() -> ()  [unwired: 2 in, 1 out]
            }
            event "CtrlRule_Description": Shortcut Menu Selection (User) {
              n210 = event-data() -> ("Type"=w318:T24, "CtlRef"=w317:refnum<vi>, "ItemTag"=w315:string)  [unwired: 1 in, 1 out]
              n211 = call "VIH UI - String Shortcut Menu Handler.vi"("Project Tree"=w316, "Menu tag"=w315, "Str Refnum"=w317, "Type"=w318) -> ()  [unwired: 8 in]
            }
            event "Comments", "CtrlRule_CtrlID", "CtrlRule_CustomName": Shortcut Menu Activation? {
              n212 = event-data() -> ("Type"=w322:T24, "CtlRef"=w321:refnum<vi>, "MenuRef"=w320:refnum<k9>)  [unwired: 1 in, 1 out]
              n213 = call "VIH UI - String Shortcut Menu Handler.vi"("Project Tree"=w319, "mode"=enum16{"basic", "format 1", "format 2"}."basic", "menu"=w320, "Str Refnum"=w321, "Type"=w322) -> ()  [unwired: 7 in]
              n214 = event-data() -> ()  [unwired: 2 in, 1 out]
            }
            event "Comments", "CtrlRule_CtrlID", "CtrlRule_CustomName": Shortcut Menu Selection (User) {
              n215 = event-data() -> ("Type"=w327:T24, "CtlRef"=w326:refnum<vi>, "ItemTag"=w324:string)  [unwired: 1 in, 1 out]
              n216 = call "VIH UI - String Shortcut Menu Handler.vi"("Project Tree"=w325, "Menu tag"=w324, "Str Refnum"=w326, "Type"=w327) -> ()  [unwired: 8 in]
            }
          }
        }
      }
      frame "STARTUP" {
        w335 = i32[] [] ("CSS List")
        w336 = 1 ("CategoryList")
        w340 = u32 16777216
        w346 = T25 {"Horizontal"=0, "Vertical"=0} ("Origin")
        w342 = T26 {"Left"=2, "Top"=0} ("Position")
        n217 = control-ref of="JS List"() -> (w339:refnum<vi>)
        n218 = control-ref of="CSS List"() -> (w338:refnum<vi>)
        n219 = control-ref of="Category List"() -> (w329:refnum<vi>)
        n220 = property on="Pane-Top" class="Pane"("Origin"=w346) -> ()  [unwired: 2 in, 2 out]
        n221 = property on="Pane-Left" class="Pane"("Origin"=w346) -> ()  [unwired: 2 in, 2 out]
        n222 = local write "Category List"(w336) -> ()
        n223 = local write "CSS List"(w335) -> ()
        n224 = Build Array(w338, w339) -> (w337:refnum<vi>[])
        n225 = property on="Pane-Right" class="Pane"("Origin"=w346) -> ("Decos[]"=w345:refnum<vi>[])  [unwired: 2 in, 2 out]
        n226 = local write "JS List"(w335) -> ()
        n227 = disable-structure shown="Disabled" {
          disable-tunnel: w337 -> [w353 _ _]
          disable-tunnel: w329 -> [_ w362 _]
          frame Disabled {
            n228 = call "VIH Utility - DEV - Get DevTime Utility VIs Folder.vi"("Utility VI Name"="Utility - Set File List Icons.vi") -> ("error out"=w358:errorcluster, "Utility VIs Path"=w357:path)  [unwired: 8 in, 1 out]
            n229 = Open VI Reference(type specifier VI Refnum (for type only)=refnum<vi> refnum, vi path=w357, error in (no error)=w358) -> (vi reference=w360:refnum<vi>, error out=w361:errorcluster)  [unwired: 3 in]
            n230 = call-by-ref "?"(reference=w360, error in=w361, "MCListbox Refnums"=w353) -> (reference out=w355:refnum<vi>, error out=w356:errorcluster, 0:"error out"=w352:errorcluster)  [unwired: 10 in]
            n231 = Close Reference(reference=w355, error in (no error)=w356) -> (error out=w351:errorcluster)
            n232 = Select(t=w351, s=w351, f=w352) -> (s? t:f=w354:errorcluster)
            n233 = call <vilib>:"Simple Error Handler.vi"("error in (no error)"=w354) -> ()  [unwired: 4 in, 5 out]
          }
          frame Disabled {
            n234 = call "VIH Utility - DEV - Get DevTime Utility VIs Folder.vi"("Utility VI Name"="Utility - Set Category List Text & Icons.vi") -> ("error out"=w370:errorcluster, "Utility VIs Path"=w369:path)  [unwired: 8 in, 1 out]
            n235 = Open VI Reference(type specifier VI Refnum (for type only)=refnum<vi> refnum, vi path=w369, error in (no error)=w370) -> (vi reference=w372:refnum<vi>, error out=w373:errorcluster)  [unwired: 3 in]
            n236 = call-by-ref "?"(reference=w372, error in=w373, "LstBox Refnum"=w362) -> (reference out=w367:refnum<vi>, error out=w368:errorcluster, 0:"error out"=w365:errorcluster)  [unwired: 10 in]
            n237 = Close Reference(reference=w367, error in (no error)=w368) -> (error out=w364:errorcluster)
            n238 = Select(t=w364, s=w364, f=w365) -> (s? t:f=w366:errorcluster)
            n239 = call <vilib>:"Simple Error Handler.vi"("error in (no error)"=w366) -> ()  [unwired: 4 in, 5 out]
          }
          frame Enabled {
          }
        }
        n240 = local write "Tab Control"(w336) -> ()
        n241 = Index Array(array=w345) -> (element=w347:refnum<vi>)  [unwired: 1 in]
        n242 = local write "CtrlRule List"(w335) -> ()
        n243 = property class="Decor"(reference=w347, "Position"=w342) -> (error out=w343:errorcluster)  [unwired: 1 in, 1 out]
        n244 = property on="Tab Control" class="TabCtl (strict)"(error in=w343, "Position"=w342, "BG Color"=w340, "FG Color"=w340, "Tabs Visible?"=FALSE, "SkipTabbing"=TRUE ("Skip When Tabbing")) -> (error out=w344:errorcluster)  [unwired: 1 in, 1 out]
        n245 = property class="VI"() -> ("FP.State"=w332:T10)  [unwired: 2 in, 2 out]
        n246 = Close Reference(reference=w345, error in (no error)=w344) -> ()  [unwired: 1 out]
        n247 = call "VIH Debug Flag Container.vi"() -> ("Debug Mode"=w334:bool)  [unwired: 11 in]
        n248 = Equal?(x=w332, y=T10."Standard" ("Front Panel Window:State")) -> (x = y?=w330:bool)
        n249 = Or(x=w330, y=w334) -> (x .or. y?=w333:bool)
        n250 = property on="%STOP" class="Bool"("Visible"=w333) -> ()  [unwired: 2 in, 2 out]
        n251 = property on="%UPDATE" class="Bool"("Visible"=w333) -> ()  [unwired: 2 in, 2 out]
      }
      frame "INIT" {
        n252 = control-ref of="MenuDscrMode"() -> (w381:refnum<vi>)
        n253 = control-ref of="VIDscrMode"() -> (w377:refnum<vi>)
        n254 = control-ref of="VIDetailsMode"() -> (w376:refnum<vi>)
        n255 = control-ref of="PVIIDscrMode"() -> (w375:refnum<vi>)
        n256 = control-ref of="Ctl_DscrMode"() -> (w374:refnum<vi>)
        n257 = Build Array(w381, w377, w376, w375, w374) -> (w378:refnum<vi>[])
        n258 = Build Array(VIH_HelpGen_Typedef_-_Enum_-_Description_Mode."Custom" ("MenuDscrMode")) -> (w379:T3[])
        n259 = for {
          tunnel: w378 -> [w385] mode=indexing
          tunnel: w379 -> [w384]
          n260 = property class="Enum (strict)"(reference=w385, "Disabled Items []"=w384) -> ()  [unwired: 1 in, 2 out]
        }
      }
      frame "EXIT" {
        w389 = i32[] [] ("Item Symbols")
        w390 = string[][] [] ("Item Names")
        w391 = T27 {"Row"=0, "Column"=0} ("Top Left Visible Cell")
        n261 = control-ref of="Tab Control"() -> (w386:refnum<vi>)
        n262 = property class="TabCtl (strict)"(reference=w386, "DisabledEnum"=T11."Enabled" ("Disabled")) -> ("Pages"=w387:refnum<vi>[])  [unwired: 1 in, 2 out]
        n263 = property on="CtrlRule List" class="MCListbox (strict)"("TopLeft"=w391, "Value"=w389, "ItemNames"=w390, "ItemSyms"=w389) -> ()  [unwired: 2 in, 2 out]
        n264 = for {
          tunnel: w387 -> [w397] mode=indexing
          n265 = property class="Page"(reference=w397) -> (reference out=w395:refnum<vi>, "Controls on Page[]"=w396:refnum<vi>[])  [unwired: 1 in, 1 out]
          n266 = for {
            tunnel: w396 -> [w401] mode=indexing
            shift-right: [w398] -> w394
            shift-left: w395 -> [w398]
            n267 = property class="Ctl"(reference=w401, "DisabledEnum"=T11."Enabled" ("Disabled")) -> (reference out=w399:refnum<vi>)  [unwired: 1 in, 1 out]
            n268 = Close Reference(reference=w399) -> ()  [unwired: 1 in, 1 out]
          }
          n269 = Close Reference(reference=w394) -> ()  [unwired: 1 in, 1 out]
        }
        n270 = property on="CSS List" class="MCListbox (strict)"("TopLeft"=w391, "Value"=w389, "ItemNames"=w390, "ItemSyms"=w389) -> ()  [unwired: 2 in, 2 out]
        n271 = property on="JS List" class="MCListbox (strict)"("TopLeft"=w391, "Value"=w389, "ItemNames"=w390, "ItemSyms"=w389) -> ()  [unwired: 2 in, 2 out]
      }
      frame "HALT" {
        w402 = TRUE ("Visible")
        w403 = u32 16777238
        n272 = Unregister For Events(event registration refnum=w410) -> (error out=w408:errorcluster)  [unwired: 1 in]
        n273 = Destroy User Event(user event=w409, error in=w408) -> (error out=w406:errorcluster)
        n274 = Release Queue(queue=w407, error in (no error)=w406) -> ()  [unwired: 1 in, 3 out]
        n275 = property on="%STOP" class="Bool"("Visible"=w402) -> ()  [unwired: 2 in, 2 out]
        n276 = property on="Tab Control" class="TabCtl (strict)"("BG Color"=w403, "FG Color"=w403, "Tabs Visible?"=TRUE) -> ()  [unwired: 2 in, 2 out]
        n277 = property on="%UPDATE" class="Bool"("Visible"=w402) -> ()  [unwired: 2 in, 2 out]
      }
      frame "------------------------------ 1" {
      }
      frame "UPDATE" {
        n278 = Unbundle(w425) -> ("Array out"=w419:string[])  [unwired: 1 out]
        n279 = case shown="Default" w418 {
          selector: w418 -> [w435 _]
          tunnel: w419 -> [_ w437]
          tunnel: [w434 w437] -> w420
          frame Default {
            n280 = call "VIH Utility - STR - String to 1D Str Array.vi"("delimiter ('\\n')"="|" ("delimiter ('\\n')"), "String in"=w435) -> ("Array out"=w434:string[])  [unwired: 5 in]
          }
          frame "REFRESH" {
          }
        }
        n281 = control-ref of="ProductInfoText"() -> (w416:refnum<vi>)
        n282 = control-ref of="Comments"() -> (w415:refnum<vi>)
        n283 = Build Array(w416, w415) -> (w417:refnum<vi>[])
        n284 = Array Size(array=w420) -> (size(s)=w422:i32)
        n285 = for {
          tunnel: w417 -> [w432] mode=indexing
          n286 = property on="Property Node" class="Str"(reference=w432, "Text.Selection"=T12 {"Selection Start"=0, "Selection End"=0}) -> ()  [unwired: 1 in, 2 out]
        }
        n287 = Greater?(x=w422, y=1) -> (0:w424:bool)
        n288 = call "VIH Utility - UI - Boolean to Control Disable Status.vi"("Status in"=w424) -> ("Control Disable if True"=w421:u8)  [unwired: 3 in, 1 out]
        n289 = property on="Tab Control" class="TabCtl (strict)"("DisabledEnum"=w421) -> ()  [unwired: 2 in, 2 out]
        n290 = Index Array(array=w420) -> (element=w426:string)  [unwired: 1 in]
        n291 = call "VIH Project - Container - Group Rules.vi"("Group ID"=w426) -> ("Group Rule out"=w427:T16)  [unwired: 6 in, 4 out]
        n292 = Bundle("Array out"=w420, "Group Rule out"=w427) -> (w428:T28)  [unwired: 1 in]
        n293 = Concatenate Strings("Update Category;\n\nSet Busy = ON;\n\nUpdate: UI;\nUpdate: Product Info;\nUpdate: General;\nUpdate: Target Paths;\nUpdate: Templates;\nUpdate: CSS List = INIT;\nUpdate: JS List = INIT;\nUpdate: Item Rules;\nUpdate: Control Rules = INIT;\n\nCSS List: Update Controls;\nJS List: Update Controls;\nCtrlRule: Update Controls = INIT;\n\nSet Busy = OFF;" ("string"), w431) -> (w430:string)
      }
      frame "Globals" {
        n294 = case shown="\"SET\"" w439 {
          tunnel: [w444 w449 w454] -> w442
          tunnel: w441 -> [w444 w448 w454]
          tunnel: w438 -> [w443 _ _]
          frame Default {
            n295 = One Button Dialog(message=w443) -> ()  [unwired: 1 in, 1 out]
          }
          frame "GET" {
            n296 = Unbundle(w448) -> ("Array out"=w446:string[])  [unwired: 1 out]
            n297 = Index Array(array=w446) -> (element=w447:string)  [unwired: 1 in]
            n298 = call "VIH Project - Container - Group Rules.vi"("Group ID"=w447) -> ("Group Rule out"=w445:T16)  [unwired: 6 in, 4 out]
            n299 = Bundle("Array out"=w446, "Group Rule out"=w445) -> (w449:T28)  [unwired: 1 in]
          }
          frame "SET" {
            n300 = Unbundle(w454) -> ("Array out"=w451:string[], "Group Rule out"=w452:T16)
            n301 = Index Array(array=w451) -> (element=w453:string)  [unwired: 1 in]
            n302 = call "VIH Project - Container - Group Rules.vi"("cmd (get)"=T13."set", "Group Rule"=w452, "Group ID"=w453) -> ()  [unwired: 4 in, 5 out]
          }
        }
      }
      frame "Update Category" {
        (unwired) "File Group"
        n303 = property on="Category List" class="LstBox (strict)"() -> ("Item Names"=w461:string[])  [unwired: 2 in, 2 out]
        n304 = Index Array(array=w461, index=w460) -> (element=w458:string)
        n305 = To Unsigned Long Integer(number=w460) -> (unsigned 32bit integer=w462:u32)
        n306 = local write "Tab Control"(w462) -> ()
        n307 = Concatenate Strings("Group Rule", " : " ("string"), w458) -> (→"CategoryTitle":string)
      }
      frame "Set Busy" {
        n308 = case shown="\"ON\"" w464 {
          frame "OFF", Default {
            n309 = call <vilib>:"Unset Busy.vi"() -> ()  [unwired: 11 in, 1 out]
          }
          frame "ON" {
            n310 = call <vilib>:"Set Busy.vi"() -> ()  [unwired: 10 in, 2 out]
          }
        }
      }
      frame "Key Focus" {
        n311 = case shown="\"CSS List\"" w468 {
          selector: w468 -> [w477 _ _ _ _ _]
          tunnel: [w477 _ _ _ _ _] -> w467
          frame Default {
          }
          frame "CtrlRule Control ID" {
            n312 = property on="CtrlRule_CtrlID" class="Str"("Key Focus"=TRUE, "Text.Selection End"=u32 9999 ("Text.Selection:End"), "Text.Selection Start"=u32 0 ("Text.Selection:Start")) -> ()  [unwired: 2 in, 2 out]
          }
          frame "CtrlRule List" {
            n313 = property on="CtrlRule List" class="MCListbox (strict)"("Key Focus"=TRUE) -> ()  [unwired: 2 in, 2 out]
          }
          frame "CSS List" {
            n314 = property on="CSS List" class="MCListbox (strict)"("Key Focus"=TRUE) -> ()  [unwired: 2 in, 2 out]
          }
          frame "JS List" {
            n315 = property on="JS List" class="MCListbox (strict)"("Key Focus"=TRUE) -> ()  [unwired: 2 in, 2 out]
          }
          frame "Category List" {
            n316 = property on="Category List" class="LstBox (strict)"("Key Focus"=TRUE) -> ()  [unwired: 2 in, 2 out]
          }
        }
        n317 = stacked-sequence {
          tunnel: w467 -> [_]
          frame #0 {
            n318 = control-ref of="CSS List"() -> (w473:refnum<vi>)
            n319 = control-ref of="JS List"() -> (w472:refnum<vi>)
            n320 = control-ref of="CtrlRule List"() -> (w471:refnum<vi>)
            n321 = control-ref of="Category List"() -> (w474:refnum<vi>)
            n322 = Build Array(w473, w472, w471) -> (w475:refnum<vi>[])
            n323 = for {
              tunnel: w475 -> [w476] mode=indexing
              n324 = call "VIH Utility - UI - Key Focus & Selection Color (MC Listbox).vi"("MCListbox Refnum"=w476) -> ()  [unwired: 8 in, 3 out]
            }
            n325 = call "VIH Utility - UI - Key Focus & Selection Color (Listbox).vi"("LstBox Refnum"=w474) -> ()  [unwired: 8 in, 3 out]
          }
        }
      }
      frame "------------------------------ 2" {
      }
      frame "Update: UI" {
        n326 = Unbundle(w489) -> ("Array out"=w488:string[])  [unwired: 1 out]
        n327 = Index Array(array=w488) -> (element=w492:string)  [unwired: 1 in]
        n328 = property class="Tree (strict)"(reference=w490, "Active Item Tag"=w492, "ActiveColNum"=0 ("Active Cell:Active Column Number")) -> ("Cell String"=w487:string)  [unwired: 1 in, 2 out]
        n329 = local write "Group Name"(w487) -> ()
      }
      frame "Update: Product Info" {
        n330 = Unbundle(w509) -> ("Group Rule out"=w508:T16)  [unwired: 1 out]
        n331 = call "VIH Project - Container - Product Info.vi"() -> ("Product Info out"=w502:T29)  [unwired: 11 in]
        n332 = Unbundle By Name(w502) -> ("ProductName"=→"PI_Product":string, "Version"=→"PI_Version":string, "Author"=→"PI_Author":string, "Company"=→"PI_Company":string, "Copyright"=→"PI_Copyright":string, "Website"=→"PI_Website":string, "Email"=→"PI_Email":string, "AddInfo"=→"PI_AddInfo":string)
        n333 = Unbundle By Name(w508) -> ("ProductInfoMode"=w505:T2, "ProductInfoText"=w503:string)
        n334 = Not Equal?(x=w505, y=VIH_HelpGen_Typedef_-_Enum_-_Default,Enable,Disable."Enable") -> (x != y?=w507:bool)
        n335 = call "VIH Utility - UI - Boolean to Control Disable Status.vi"("Status in"=w507) -> ("Control Disable if True"=w504:u8)  [unwired: 3 in, 1 out]
        n336 = property on="ProductInfoMode" class="Ring (strict)"("Value"=w505) -> ()  [unwired: 2 in, 2 out]
        n337 = property on="ProductInfoText" class="Str"("DisabledEnum"=w504, "Value"=w503) -> ()  [unwired: 2 in, 2 out]
      }
      frame "Update: General" {
        n338 = Unbundle(w518) -> ("Group Rule out"=w517:T16)  [unwired: 1 out]
        n339 = Unbundle By Name(w517) -> ("BuildHelp"=w516:T2, "Flags"=w515:T21, "%Comments"=w511:string)
        n340 = Unbundle By Name(w515) -> ("Override CSS Files"=w514:bool, "Override JS Files"=w513:bool, "Override Ctl Rules"=w512:bool)
        n341 = local write "BuildHelp"(w516) -> ()
        n342 = local write "Comments"(w511) -> ()
        n343 = local write "Override_CSS Files"(w514) -> ()
        n344 = local write "Override_JS Files"(w513) -> ()
        n345 = local write "Override_Ctl Rules"(w512) -> ()
      }
      frame "Update: Target Paths" {
        w520 = FALSE ("Allow Empty Path (T)")
        w521 = TRUE ("Ena Empty Path")
        n346 = Unbundle(w562) -> ("Array out"=w534:string[], "Group Rule out"=w561:T16)
        n347 = Index Array(array=w534) -> (element=w533:string)  [unwired: 1 in]
        n348 = Unbundle By Name(w561) -> ("Target Paths"=w560:T18)
        n349 = call "VIH Project - Get Effective Group Rule.vi"("Ignore Control Rules (F)"=TRUE, "Group ID"=w533, "Project Tree"=w535) -> ("Effective Group Rule"=w531:T16)  [unwired: 6 in, 2 out]
        n350 = Unbundle By Name(w560) -> ("HTML Dir"=w559:path, "Image Dir"=w552:path, "CSS Dir"=w553:path, "JS Dir"=w554:path)
        n351 = Unbundle By Name(w531) -> ("Build Root Dir"=w526:path)
        "Build Root Dir" <- w526
        n352 = Unbundle By Name(w531) -> ("Target Paths.HTML Dir"=w545:path, "Target Paths.Image Dir"=w538:path, "Target Paths.CSS Dir"=w537:path, "Target Paths.JS Dir"=w536:path)
        n353 = call "VIH UI - Path Indication (with Default).vi"("Ena Empty Path"=w521, "Path"=w553) -> ("Custom"=w541:bool, "Disable"=w556:u8, "Path out"=w542:path)  [unwired: 7 in]
        n354 = call "VIH UI - Path Indication (with Default).vi"("Ena Empty Path"=w521, "Path"=w554) -> ("Custom"=w539:bool, "Disable"=w555:u8, "Path out"=w540:path)  [unwired: 7 in]
        n355 = call "VIH UI - Path Indication (with Default).vi"("Ena Empty Path"=w521, "Path"=w552) -> ("Custom"=w543:bool, "Disable"=w557:u8, "Path out"=w544:path)  [unwired: 7 in]
        n356 = call "VIH UI - Path Indication (with Default).vi"("Ena Empty Path"=w521, "Path"=w559) -> ("Custom"=w546:bool, "Disable"=w558:u8, "Path out"=w547:path)  [unwired: 7 in]
        n357 = Boolean To (0,1)(Boolean=w543) -> (0, 1=w550:i16)
        n358 = Select(t=w547, s=w546, f=w545) -> (s? t:f=w522:path)
        n359 = Boolean To (0,1)(Boolean=w541) -> (0, 1=w549:i16)
        n360 = Boolean To (0,1)(Boolean=w539) -> (0, 1=w548:i16)
        n361 = Select(t=w540, s=w539, f=w536) -> (s? t:f=w525:path)
        n362 = Boolean To (0,1)(Boolean=w546) -> (0, 1=w551:i16)
        n363 = Select(t=w544, s=w543, f=w538) -> (s? t:f=w523:path)
        n364 = Select(t=w542, s=w541, f=w537) -> (s? t:f=w524:path)
        n365 = call "VIH HelpGen - FILE - Build Absolute Path.vi"("Root Path"=w526, "Allow Empty Path (T)"=w520, "Path in"=w522) -> ("Path out"=w527:path)  [unwired: 8 in]
        n366 = call "VIH HelpGen - FILE - Build Absolute Path.vi"("Root Path"=w526, "Allow Empty Path (T)"=w520, "Path in"=w523) -> ("Path out"=w528:path)  [unwired: 8 in]
        n367 = call "VIH HelpGen - FILE - Build Absolute Path.vi"("Root Path"=w526, "Allow Empty Path (T)"=w520, "Path in"=w524) -> ("Path out"=w529:path)  [unwired: 8 in]
        n368 = call "VIH HelpGen - FILE - Build Absolute Path.vi"("Root Path"=w526, "Allow Empty Path (T)"=w520, "Path in"=w525) -> ("Path out"=w530:path)  [unwired: 8 in]
        n369 = property on="Dst_HTML Dir" class="Path"("Value"=w522, "DisabledEnum"=w558, "StartPath"=w527) -> ()  [unwired: 2 in, 2 out]
        n370 = local write "Custom_HTML Dir"(w551) -> ()
        n371 = property on="Dst_Image Dir" class="Path"("Value"=w523, "DisabledEnum"=w557, "StartPath"=w528) -> ()  [unwired: 2 in, 2 out]
        n372 = local write "Custom_Image Dir"(w550) -> ()
        n373 = property on="Dst_CSS Dir" class="Path"("Value"=w524, "DisabledEnum"=w556, "StartPath"=w529) -> ()  [unwired: 2 in, 2 out]
        n374 = local write "Custom_CSS Dir"(w549) -> ()
        n375 = property on="Dst_JS Dir" class="Path"("Value"=w525, "DisabledEnum"=w555, "StartPath"=w530) -> ()  [unwired: 2 in, 2 out]
        n376 = local write "Custom_JS Dir"(w548) -> ()
      }
      frame "Update: Templates" {
        n377 = Unbundle(w601) -> ("Array out"=w576:string[], "Group Rule out"=w600:T16)
        n378 = Index Array(array=w576) -> (element=w575:string)  [unwired: 1 in]
        n379 = call "VIH Project - Get Effective Group Rule.vi"("Ignore Control Rules (F)"=TRUE, "Group ID"=w575, "Project Tree"=w578) -> ("Effective Group Rule"=w574:T16)  [unwired: 6 in, 2 out]
        n380 = Unbundle By Name(w574) -> ("Source Paths.VI Template"=w582:path, "Source Paths.Menu Template"=w581:path, "Source Paths.PolyVI Template"=w565:path)
        n381 = Unbundle By Name(w600) -> ("Source Paths"=w599:T17)
        n382 = Unbundle By Name(w599) -> ("VI Template"=w596:path, "Menu Template"=w586:path, "PolyVI Template"=w564:path)
        n383 = call "VIH UI - Path Indication (with Default).vi"("Ena Empty Path"=FALSE, "Path"=w596) -> ("Custom"=w592:bool, "Disable"=w593:u8, "Path out"=w595:path)  [unwired: 7 in]
        n384 = call "VIH UI - Path Indication (with Default).vi"("Ena Empty Path"=FALSE, "Path"=w586) -> ("Custom"=w587:bool, "Disable"=w589:u8, "Path out"=w588:path)  [unwired: 7 in]
        n385 = call "VIH UI - Path Indication (with Default).vi"("Ena Empty Path"=FALSE, "Path"=w564) -> ("Custom"=w569:bool, "Disable"=w567:u8, "Path out"=w568:path)  [unwired: 7 in]
        n386 = case shown="True" w592 {
          tunnel: [w613 w617] -> w598
          tunnel: [_ w616] -> w597
          tunnel: w595 -> [_ w615]
          tunnel: [w614 _] -> w594
          tunnel: w593 -> [w614 _]
          tunnel: w582 -> [w613 _]
          frame False {
          }
          frame True {
            n387 = call "VIH UI - Test Path.vi"("Path"=w615) -> ("Color"=w616:u32, "dup Path"=w617:path)  [unwired: 7 in, 2 out]
          }
        }
        n388 = case shown="True" w587 {
          tunnel: [w608 w612] -> w585
          tunnel: [_ w611] -> w583
          tunnel: w588 -> [_ w610]
          tunnel: [w609 _] -> w584
          tunnel: w589 -> [w609 _]
          tunnel: w581 -> [w608 _]
          frame False {
          }
          frame True {
            n389 = call "VIH UI - Test Path.vi"("Path"=w610) -> ("Color"=w611:u32, "dup Path"=w612:path)  [unwired: 7 in, 2 out]
          }
        }
        n390 = case shown="True" w569 {
          tunnel: [w603 w607] -> w570
          tunnel: [_ w606] -> w572
          tunnel: w568 -> [_ w605]
          tunnel: [w604 _] -> w571
          tunnel: w567 -> [w604 _]
          tunnel: w565 -> [w603 _]
          frame False {
          }
          frame True {
            n391 = call "VIH UI - Test Path.vi"("Path"=w605) -> ("Color"=w606:u32, "dup Path"=w607:path)  [unwired: 7 in, 2 out]
          }
        }
        n392 = Boolean To (0,1)(Boolean=w592) -> (0, 1=w580:i16)
        n393 = Boolean To (0,1)(Boolean=w587) -> (0, 1=w579:i16)
        n394 = Boolean To (0,1)(Boolean=w569) -> (0, 1=w573:i16)
        n395 = property on="Src_VI Template" class="Path"("Value"=w598, "Text.TextColor"=w597, "DisabledEnum"=w594) -> ()  [unwired: 2 in, 2 out]
        n396 = local write "Custom_VI Template"(w580) -> ()
        n397 = property on="Src_Menu Template" class="Path"("Value"=w585, "Text.TextColor"=w583, "DisabledEnum"=w584) -> ()  [unwired: 2 in, 2 out]
        n398 = property on="Src_PolyVI Template" class="Path"("Value"=w570, "Text.TextColor"=w572, "DisabledEnum"=w571) -> ()  [unwired: 2 in, 2 out]
        n399 = local write "Custom_PolyVI Template"(w573) -> ()
        n400 = local write "Custom_Menu Template"(w579) -> ()
      }
      frame "Update: CSS List" {
        n401 = Unbundle(w635) -> ("Group Rule out"=w634:T16)  [unwired: 1 out]
        n402 = Unbundle By Name(w634) -> ("Source Paths"=w633:T17)
        n403 = Unbundle By Name(w633) -> ("CSS Files"=w624:path[])
        n404 = Array Size(array=w624) -> (size(s)=w623:i32)
        n405 = for {
          tunnel: w624 -> [w642] mode=indexing
          tunnel: [w641] -> w619 mode=indexing
          tunnel: [w643] -> w632 mode=indexing
          n406 = Path To String(path=w642) -> (string=w644:string)
          n407 = call "VIH UI - Test Path.vi"("Path"=w642) -> ("Symbol"=w641:i32)  [unwired: 7 in, 3 out]
          n408 = Build Array(w644) -> (w643:string[])
        }
        n409 = Not Equal?(x=w619, y=0) -> (x != y?=w621:bool[])
        n410 = call "VIH Utility - UI - Drag and Drop Supporter (w Symbol Indices).vi"("Cmd"=enum16{"make symbols", "test D'n'D"}."make symbols", "Item Symbols"=w619) -> ("Item Symbols out"=w630:i32[])  [unwired: 7 in, 2 out]
        n411 = Or Array Elements(Boolean array=w621) -> (logical OR=w618:bool)
        n412 = control-ref of="CSS List"() -> (w629:refnum<vi>)
        n413 = property on="CSS List" class="MCListbox (strict)"("ItemNames"=w632, "ItemSyms"=w630, "Symbols Vis"=w618) -> (error out=w622:errorcluster)  [unwired: 2 in, 1 out]
        n414 = case shown="\"INIT\"" w625 {
          tunnel: w623 -> [_ w640]
          tunnel: w627 -> [w637 w639]
          tunnel: [w637 w638] -> w626
          tunnel: w622 -> [_ _]
          frame Default {
          }
          frame "INIT" {
            n415 = call "VIH UI - Coerce List Value.vi"("# elements"=w640, "Indices in"=w639) -> ("Indices out"=w638:i32[])  [unwired: 9 in]
            n416 = property on="CSS List" class="MCListbox (strict)"("Value"=w638) -> ()  [unwired: 2 in, 2 out]
          }
        }
        n417 = Index Array(array=w626) -> (element=w628:i32)  [unwired: 1 in]
        n418 = call "VIH Utility - UI - Make Row Visible (MC Listbox).vi"("Row"=w628, "MC Listbox Refnum"=w629) -> ()  [unwired: 8 in, 2 out]
      }
      frame "Update: JS List" {
        n419 = Unbundle(w662) -> ("Group Rule out"=w661:T16)  [unwired: 1 out]
        n420 = Unbundle By Name(w661) -> ("Source Paths"=w660:T17)
        n421 = Unbundle By Name(w660) -> ("JS Files"=w652:path[])
        n422 = Array Size(array=w652) -> (size(s)=w651:i32)
        n423 = for {
          tunnel: w652 -> [w669] mode=indexing
          tunnel: [w668] -> w646 mode=indexing
          tunnel: [w670] -> w659 mode=indexing
          n424 = Path To String(path=w669) -> (string=w671:string)
          n425 = call "VIH UI - Test Path.vi"("Path"=w669) -> ("Symbol"=w668:i32)  [unwired: 7 in, 3 out]
          n426 = Build Array(w671) -> (w670:string[])
        }
        n427 = Not Equal?(x=w646, y=0) -> (x != y?=w648:bool[])
        n428 = Or Array Elements(Boolean array=w648) -> (logical OR=w645:bool)
        n429 = call "VIH Utility - UI - Drag and Drop Supporter (w Symbol Indices).vi"("Cmd"=enum16{"make symbols", "test D'n'D"}."make symbols", "Item Symbols"=w646) -> ("Item Symbols out"=w657:i32[])  [unwired: 7 in, 2 out]
        n430 = control-ref of="JS List"() -> (w655:refnum<vi>)
        n431 = property on="JS List" class="MCListbox (strict)"("ItemNames"=w659, "ItemSyms"=w657, "Symbols Vis"=w645) -> (error out=w649:errorcluster)  [unwired: 2 in, 1 out]
        n432 = case shown="\"INIT\"" w654 {
          tunnel: w651 -> [_ w667]
          tunnel: w653 -> [w664 w666]
          tunnel: [w664 w665] -> w650
          tunnel: w649 -> [_ _]
          frame Default {
          }
          frame "INIT" {
            n433 = call "VIH UI - Coerce List Value.vi"("# elements"=w667, "Indices in"=w666) -> ("Indices out"=w665:i32[])  [unwired: 9 in]
            n434 = property on="JS List" class="MCListbox (strict)"("Value"=w665) -> ()  [unwired: 2 in, 2 out]
          }
        }
        n435 = Index Array(array=w650) -> (element=w656:i32)  [unwired: 1 in]
        n436 = call "VIH Utility - UI - Make Row Visible (MC Listbox).vi"("Row"=w656, "MC Listbox Refnum"=w655) -> ()  [unwired: 8 in, 2 out]
      }
      frame "Update: Item Rules" {
        n437 = Unbundle(w681) -> ("Group Rule out"=w677:T16)  [unwired: 1 out]
        n438 = Unbundle By Name(w677) -> ("VIDscrMode"=w680:T3, "MenuDscrMode"=w679:T3, "MenuItemIcons"=w678:T2, "PVIIDscrMode"=w673:T3, "VIDetailsMode"=w672:T3)
        n439 = Unbundle By Name(w677) -> ("Ctl_DscrMode"=w676:T3, "Ctl_ClustMembers"=w675:T2, "Ctl_EnumValues"=w674:T2)
        n440 = local write "VIDscrMode"(w680) -> ()
        n441 = local write "MenuDscrMode"(w679) -> ()
        n442 = local write "MenuItemIcons"(w678) -> ()
        n443 = local write "PVIIDscrMode"(w673) -> ()
        n444 = local write "VIDetailsMode"(w672) -> ()
        n445 = local write "Ctl_DscrMode"(w676) -> ()
        n446 = local write "Ctl_ClustMembers"(w675) -> ()
        n447 = local write "Ctl_EnumValues"(w674) -> ()
      }
      frame "Update: Control Rules" {
        n448 = Unbundle(w696) -> ("Group Rule out"=w695:T16)  [unwired: 1 out]
        n449 = Unbundle By Name(w695) -> ("Control Rules"=w688:T19[])
        n450 = Array Size(array=w688) -> (size(s)=w687:i32)
        n451 = for {
          tunnel: w688 -> [w713] mode=indexing
          tunnel: [w711] -> w694 mode=indexing
          tunnel: [w707] -> w693 mode=indexing
          n452 = Unbundle By Name(w713) -> ("CtrlID"=w712:string, "CustomRule"=w710:bool, "EnumValDscr"=w703:T20[])
          n453 = Empty Array?(array=w703) -> (empty?=w706:bool)
          n454 = Select(t="", s=w706, f="VList") -> (s? t:f=w702:string)
          n455 = Select(t=38, s=w710, f=37) -> (s? t:f=w707:i32)
          n456 = Build Array(w712, w702) -> (w711:string[])
        }
        n457 = call "VIH Utility - UI - Drag and Drop Supporter (w Symbol Indices).vi"("Cmd"=enum16{"make symbols", "test D'n'D"}."make symbols", "Item Symbols"=w693) -> ("Item Symbols out"=w692:i32[])  [unwired: 7 in, 2 out]
        n458 = control-ref of="CtrlRule List"() -> (w690:refnum<vi>)
        n459 = property on="CtrlRule List" class="MCListbox (strict)"("ItemNames"=w694, "ItemSyms"=w692) -> (error out=w683:errorcluster)  [unwired: 2 in, 1 out]
        n460 = case shown="\"INIT\"" w684 {
          tunnel: w687 -> [_ w701]
          tunnel: w686 -> [w698 w700]
          tunnel: [w698 w699] -> w685
          tunnel: w683 -> [_ _]
          frame Default {
          }
          frame "INIT" {
            n461 = call "VIH UI - Coerce List Value.vi"("# elements"=w701, "Indices in"=w700) -> ("Indices out"=w699:i32[])  [unwired: 9 in]
            n462 = property on="CtrlRule List" class="MCListbox (strict)"("Value"=w699) -> ()  [unwired: 2 in, 2 out]
          }
        }
        n463 = Index Array(array=w685) -> (element=w689:i32)  [unwired: 1 in]
        n464 = call "VIH Utility - UI - Make Row Visible (MC Listbox).vi"("Row"=w689, "MC Listbox Refnum"=w690) -> ()  [unwired: 8 in, 2 out]
      }
      frame "------------------------------ 3" {
      }
      frame "Apply: UI" {
        w716 = FALSE  # Set Focus
        n465 = Unbundle(w721) -> ("Array out"=w725:string[])  [unwired: 1 out]
        n466 = call <vilib>:"Trim Whitespace.vi"("string"="Group Name") -> ("trimmed string"=w723:string)  [unwired: 1 in]
        n467 = Index Array(array=w725) -> (element=w718:string)  [unwired: 1 in]
        n468 = Empty String/Path?(string/path=w723) -> (empty?=w724:bool)
        n469 = Select(t="Group", s=w724, f=w723) -> (s? t:f=w717:string)
        n470 = call "VIH Project Tree - Rename Item.vi"("Set Focus (T)"=w716, "New Item Name"=w717, "Item Tag"=w718, "Project Tree"=w719) -> ()  [unwired: 5 in, 3 out]
      }
      frame "Apply: Product Info" {
        n471 = Unbundle(w734) -> ("Array out"=w733:string[], "Group Rule out"=w731:T16)
        n472 = in-place {
          n473 = in-place-cluster #1(w731) -> ("ProductInfoMode"=w735:T2)  [unwired: 1 out]
          n474 = Type Cast(type=w735, x="ProductInfoMode") -> (*(type *) &x=w736:T2)
          n475 = in-place-cluster #1("ProductInfoMode"=w736, "ProductInfoText"="ProductInfoText") -> (w730:T16)
        }
        n476 = Concatenate Strings("Globals = Set;\n\nUpdate: Product Info;" ("string"), w728) -> (w727:string)
        n477 = Bundle("Array out"=w733, "Group Rule out"=w730) -> (w732:T28)  [unwired: 1 in]
      }
      frame "Apply: General" {
        n478 = Unbundle(w745) -> ("Array out"=w744:string[], "Group Rule out"=w742:T16)
        n479 = in-place {
          w751 = path ""
          n480 = in-place-cluster #2(w742) -> ()  [unwired: 7 out]
          n481 = in-place-cluster #2("Source Root Dir"=w751, "Build Root Dir"=w751, "BuildHelp"="BuildHelp", "Flags.Override CSS Files"="Override_CSS Files", "Flags.Override JS Files"="Override_JS Files", "Flags.Override Ctl Rules"="Override_Ctl Rules", "%Comments"="Comments") -> (w741:T16)
        }
        n482 = Concatenate Strings("Globals = Set;" ("string"), w746) -> (w740:string)
        n483 = Bundle("Array out"=w744, "Group Rule out"=w741) -> (w743:T28)  [unwired: 1 in]
      }
      frame "Apply: Target Paths" {
        n484 = Unbundle(w760) -> ("Array out"=w759:string[], "Group Rule out"=w757:T16)
        n485 = in-place {
          n486 = in-place-cluster #3(w757) -> ()  [unwired: 4 out]
          n487 = call "VIH Constant - Default Path Keyword.vi"() -> ("<default> path"=w761:path)  [unwired: 11 in]
          n488 = Greater Than 0?(x="Custom_Image Dir") -> (x > 0?=w776:bool)
          n489 = Greater Than 0?(x="Custom_HTML Dir") -> (x > 0?=w777:bool)
          n490 = Greater Than 0?(x="Custom_CSS Dir") -> (x > 0?=w775:bool)
          n491 = Greater Than 0?(x="Custom_JS Dir") -> (x > 0?=w774:bool)
          n492 = Select(t="Dst_Image Dir", s=w776, f=w761) -> (s? t:f=w764:path)
          n493 = Select(t="Dst_HTML Dir", s=w777, f=w761) -> (s? t:f=w765:path)
          n494 = Select(t="Dst_CSS Dir", s=w775, f=w761) -> (s? t:f=w763:path)
          n495 = Select(t="Dst_JS Dir", s=w774, f=w761) -> (s? t:f=w762:path)
          n496 = in-place-cluster #3("Target Paths.HTML Dir"=w765, "Target Paths.Image Dir"=w764, "Target Paths.CSS Dir"=w763, "Target Paths.JS Dir"=w762) -> (w756:T16)
        }
        n497 = Concatenate Strings("Globals = Set;\n\nUpdate: Target Paths;" ("string"), w754) -> (w753:string)
        n498 = Bundle("Array out"=w759, "Group Rule out"=w756) -> (w758:T28)  [unwired: 1 in]
      }
      frame "Apply: Templates" {
        n499 = Unbundle(w785) -> ("Array out"=w784:string[], "Group Rule out"=w782:T16)
        n500 = in-place {
          n501 = in-place-cluster #4(w782) -> ()  [unwired: 3 out]
          n502 = call "VIH Project - Container - Project File Path.vi"() -> ("Project File Path"=w787:path)  [unwired: 9 in, 2 out]
          n503 = Strip Path(path=w787) -> (stripped path=w786:path)  [unwired: 1 out]
          n504 = call "VIH HelpGen - FILE - Build Absolute Path.vi"("Root Path"=w786, "Allow Empty Path (T)"=TRUE, "Path in"="Src_VI Template") -> ("Path out"=w792:path)  [unwired: 8 in]
          n505 = call "VIH HelpGen - FILE - Build Absolute Path.vi"("Root Path"=w786, "Allow Empty Path (T)"=TRUE, "Path in"="Src_Menu Template") -> ("Path out"=w790:path)  [unwired: 8 in]
          n506 = call "VIH HelpGen - FILE - Build Absolute Path.vi"("Root Path"=w786, "Allow Empty Path (T)"=TRUE, "Path in"="Src_PolyVI Template") -> ("Path out"=w788:path)  [unwired: 8 in]
          n507 = call "VIH Constant - Default Path Keyword.vi"() -> ("<default> path"=w798:path)  [unwired: 11 in]
          n508 = Greater Than 0?(x="Custom_VI Template") -> (x > 0?=w802:bool)
          n509 = Greater Than 0?(x="Custom_Menu Template") -> (x > 0?=w801:bool)
          n510 = Greater Than 0?(x="Custom_PolyVI Template") -> (x > 0?=w800:bool)
          n511 = Select(t=w792, s=w802, f=w798) -> (s? t:f=w804:path)
          n512 = Select(t=w790, s=w801, f=w798) -> (s? t:f=w803:path)
          n513 = Select(t=w788, s=w800, f=w798) -> (s? t:f=w797:path)
          n514 = in-place-cluster #4("Source Paths.VI Template"=w804, "Source Paths.Menu Template"=w803, "Source Paths.PolyVI Template"=w797) -> (w781:T16)
        }
        n515 = Concatenate Strings("Globals = Set;\n\nUpdate: Templates;" ("string"), w779) -> (w778:string)
        n516 = Bundle("Array out"=w784, "Group Rule out"=w781) -> (w783:T28)  [unwired: 1 in]
      }
      frame "Apply: Item Rules" {
        n517 = Unbundle(w814) -> ("Array out"=w813:string[], "Group Rule out"=w811:T16)
        n518 = in-place {
          n519 = in-place-cluster #5(w811) -> ()  [unwired: 8 out]
          n520 = in-place-cluster #5("VIDscrMode"="VIDscrMode", "MenuDscrMode"="MenuDscrMode", "MenuItemIcons"="MenuItemIcons", "Ctl_DscrMode"="Ctl_DscrMode", "Ctl_ClustMembers"="Ctl_ClustMembers", "Ctl_EnumValues"="Ctl_EnumValues", "PVIIDscrMode"="PVIIDscrMode", "VIDetailsMode"="VIDetailsMode") -> (w810:T16)
        }
        n521 = Concatenate Strings("Globals = Set;" ("string"), w808) -> (w807:string)
        n522 = Bundle("Array out"=w813, "Group Rule out"=w810) -> (w812:T28)  [unwired: 1 in]
      }
      frame "------------------------------ 4" {
      }
      frame "CtrlRule: Update Controls" {
        n523 = Unbundle(w841) -> ("Group Rule out"=w840:T16)  [unwired: 1 out]
        n524 = Array Size(array=w831) -> (size(s)=w830:i32)
        n525 = Index Array(array=w831) -> (element=w828:i32)  [unwired: 1 in]
        n526 = Unbundle By Name(w840) -> ("Control Rules"=w839:T19[])
        n527 = case shown="\"INIT\"" w825 {
          frame Default {
          }
          frame "INIT" {
            n528 = control-ref of="CtrlRule_CtrlID"() -> (w845:refnum<vi>)
            n529 = control-ref of="CtrlRule_CustomName"() -> (w844:refnum<vi>)
            n530 = control-ref of="CtrlRule_Description"() -> (w843:refnum<vi>)
            n531 = Build Array(w845, w844, w843) -> (w846:refnum<vi>[])
            n532 = for {
              tunnel: w846 -> [w847] mode=indexing
              n533 = property on="Property Node" class="Str"(reference=w847, "Text.Selection"=T12 {"Selection Start"=0, "Selection End"=0}) -> ()  [unwired: 1 in, 2 out]
            }
          }
        }
        n534 = case shown="1" w830 {
          tunnel: w828 -> [_ w862 _]
          tunnel: w839 -> [_ w861 _]
          tunnel: [_ w859 _] -> w838
          tunnel: [_ w858 _] -> w837
          tunnel: [_ w854 _] -> w836
          tunnel: [_ w857 _] -> w835
          tunnel: [_ w856 _] -> w834
          tunnel: [_ w855 _] -> w833
          tunnel: [w849 _ w863] -> w826
          tunnel: [w849 w852 w863] -> w832
          tunnel: [w849 _ _] -> w829
          tunnel: [_ w850 _] -> w827
          frame ..0 {
            w849 = u8 2
          }
          frame 1 {
            n535 = Index Array(array=w861, index=w862) -> (element=w860:T19)
            n536 = Unbundle By Name(w860) -> ("CtrlID"=w859:string, "CustomRule"=w858:bool, "DscrMode"=w854:T3, "Description"=w857:string, "ClusterMembers"=w856:T2, "EnumValues"=w855:T2, "CustomName"=w850:string)
            n537 = Equal?(x=VIH_HelpGen_Typedef_-_Enum_-_Description_Mode."Custom", y=w854) -> (x = y?=w851:bool)
            n538 = call "VIH Utility - UI - Boolean to Control Disable Status.vi"("Status in"=w851) -> ("Control Disable if False"=w852:u8)  [unwired: 3 in, 1 out]
          }
          frame 2.. {
            w863 = u8 2
          }
        }
        n539 = property on="%CtrlRule_Copy" class="Bool"("DisabledEnum"=w829) -> ()  [unwired: 2 in, 2 out]
        n540 = property on="CtrlRule_CtrlID" class="Str"("DisabledEnum"=w826, "Value"=w838) -> ()  [unwired: 2 in, 2 out]
        n541 = property on="CtrlRule_DscrMode" class="Enum (strict)"("DisabledEnum"=w826, "Value"=w836) -> ()  [unwired: 2 in, 2 out]
        n542 = property on="CtrlRule_ClusterMembers" class="Enum (strict)"("DisabledEnum"=w826, "Value"=w834) -> ()  [unwired: 2 in, 2 out]
        n543 = property on="CtrlRule_CustomName" class="Str"("DisabledEnum"=w826, "Value"=w827) -> ()  [unwired: 2 in, 2 out]
        n544 = property on="CtrlRule_CustomRule" class="Bool (strict)"("DisabledEnum"=w826, "Value"=w837) -> ()  [unwired: 2 in, 2 out]
        n545 = property on="CtrlRule_Description" class="Str"("DisabledEnum"=w832, "Value"=w835) -> ()  [unwired: 2 in, 2 out]
        n546 = property on="CtrlRule_EnumValues" class="Enum (strict)"("DisabledEnum"=w826, "Value"=w833) -> ()  [unwired: 2 in, 2 out]
        n547 = property on="%CtrlRule_Remove" class="Bool"("DisabledEnum"=w829) -> ()  [unwired: 2 in, 2 out]
        n548 = property on="%CtrlRule_Edit_Enum" class="Bool"("DisabledEnum"=w826) -> ()  [unwired: 2 in, 2 out]
      }
      frame "CtrlRule: Add" {
        n549 = Unbundle(w874) -> ("Group Rule out"=w876:T16)  [unwired: 1 out]
        n550 = Array Size(array=w866) -> (size(s)=w870:i32)
        n551 = Array Max & Min(array=w866) -> (max value=w868:i32)  [unwired: 3 out]
        n552 = Less Or Equal To 0?(x=w870) -> (x <= 0?=w869:bool)
        n553 = Select(t=-1, s=w869, f=w868) -> (s? t:f=w865:i32)
        n554 = Increment(x=w865) -> (x+1=w864:i32)
        n555 = in-place {
          in-place-border: w864 -> [w878]
          n556 = in-place-cluster #6(w876) -> ("Control Rules"=w886:T19[])
          n557 = Array Size(array=w886) -> (size(s)=w887:i32)
          n558 = Index Array(array=w886, index=-1 ("f")) -> (element=w885:T19)
          n559 = In Range and Coerce(upper limit=w887, x=w878, lower limit=0) -> (coerced(x)=w883:i32)  [unwired: 1 out]
          n560 = Bundle By Name(cluster=w885, "CtrlID"="<Control Name>", "CustomRule"=TRUE) -> (w884:T19)
          n561 = Build Array(w883) -> (w882:i32[])
          n562 = local write "CtrlRule List"(w882) -> ()
          n563 = Insert Into Array(array=w886, index=w883, new element=w884) -> (w889:T19[])
          n564 = in-place-cluster #6("Control Rules"=w889) -> (w875:T16)
        }
        n565 = Concatenate Strings("Globals = Set;\n\nUpdate: Control Rules;\nCtrlRule: Update Controls = INIT;" ("string"), w877) -> (w872:string)
        n566 = Bundle(cluster=w874, "Group Rule out"=w875) -> (w873:T28)  [unwired: 1 in]
      }
      frame "CtrlRule: Import" {
        n567 = case shown="\"VI\", Default" w894 {
          tunnel: [w912 w920] -> w895
          tunnel: [TRUE w919] -> w893
          tunnel: w892 -> [w905 _]
          tunnel: [w902 -1 ("t")] -> w891
          tunnel: w890 -> [_ w916]
          frame "CB", "Clipboard" {
            n568 = invoke class="App" method="Clipboard.Read"() -> ("Read Clipbrd"=w911:string)  [unwired: 3 in, 2 out]
            n569 = Array Size(array=w905) -> (size(s)=w908:i32)
            n570 = Array Max & Min(array=w905) -> (max value=w903:i32)  [unwired: 3 out]
            n571 = Less Or Equal To 0?(x=w908) -> (x <= 0?=w907:bool)
            n572 = Select(t=-1, s=w907, f=w903) -> (s? t:f=w904:i32)
            n573 = call "VIH XML - Control Rules to-from XML String.vi"("cmd (check)"=enum16{"check", "parse", "format"}."parse", "XML in"=w911) -> ("Control Rules out"=w912:T19[])  [unwired: 6 in, 3 out]
            n574 = Increment(x=w904) -> (x+1=w902:i32)
          }
          frame "VI", Default {
            n575 = call "VIH Dialog - Project File List.vi"("Ena Custom VI (F)"=TRUE, "File set (All)"=enum32{"ALL", "conpane", "invalid"}."conpane", "Project Tree"=w916) -> ("OK out"=w915:bool, "File Path"=w917:path)  [unwired: 6 in, 1 out]
            n576 = case shown="True" w915 {
              tunnel: w917 -> [_ w924]
              tunnel: [_ w923] -> w919
              tunnel: [_ w922] -> _
              tunnel: [_ w921] -> w920
              frame False {
              }
              frame True {
                n577 = call "VIH Dialog - VI Terminals.vi"("VI Path"=w924) -> ("OK out"=w923:bool, "Ctrl Rules"=w921:T19[], "Ctrl IDs out"=w922:string[])  [unwired: 7 in, 1 out]
              }
            }
          }
        }
        n578 = Empty Array?(array=w895) -> (empty?=w896:bool)
        n579 = case shown="False" w896 {
          tunnel: w900 -> [w929 w938]
          tunnel: [w928 w938] -> w898
          tunnel: ["Globals = Set;\n\nUpdate: Control Rules;\nCtrlRule: Update Controls = INIT;" ("string") _] -> w897
          tunnel: w895 -> [w926 _]
          tunnel: w893 -> [_ w937]
          tunnel: w891 -> [w925 _]
          frame False {
            n580 = Unbundle(w929) -> ("Group Rule out"=w931:T16)  [unwired: 1 out]
            n581 = in-place {
              in-place-border: w926 -> [w934]
              in-place-border: w925 -> [w932]
              n582 = in-place-cluster #7(w931) -> ("Control Rules"=w936:T19[])
              n583 = call "VIH UI - Append Control Rules.vi"("Position Index (-1)"=w932, "Ctrl Rules (new)"=w934, "Ctrl Rules (existing)"=w936) -> ("Indices"=w933:i32[], "Ctrl Rules out"=w935:T19[])  [unwired: 7 in]
              n584 = in-place-cluster #7("Control Rules"=w935) -> (w930:T16)
              n585 = property on="CtrlRule List" class="MCListbox (strict)"("Value"=w933) -> ()  [unwired: 2 in, 2 out]
            }
            n586 = Bundle(cluster=w929, "Group Rule out"=w930) -> (w928:T28)  [unwired: 1 in]
          }
          frame True {
            n587 = case shown="True" w937 {
              frame False {
              }
              frame True {
                n588 = call <vilib>:"Beep.vi"() -> ()  [unwired: 12 in]
              }
            }
          }
        }
        n589 = Concatenate Strings(w897, w901) -> (w899:string)
      }
      frame "CtrlRule: Export" {
        n590 = Unbundle(w945) -> ("Group Rule out"=w947:T16)  [unwired: 1 out]
        n591 = Unbundle By Name(w947) -> ("Control Rules"=w944:T19[])
        n592 = for {
          tunnel: w946 -> [w951] mode=indexing
          tunnel: w944 -> [w950]
          tunnel: [w949] -> w939 mode=indexing
          n593 = Index Array(array=w950, index=w951) -> (element=w949:T19)
        }
        n594 = call "VIH XML - Control Rules to-from XML String.vi"("cmd (check)"=enum16{"check", "parse", "format"}."format", "Control Rules in"=w939) -> ("error out"=w942:errorcluster, "XML out"=w941:string)  [unwired: 6 in, 2 out]
        n595 = invoke class="App" method="Clipboard.Write"(error in=w942, "Param 0"=w941) -> (error out=w940:errorcluster)  [unwired: 2 in, 3 out]
        n596 = call <vilib>:"Simple Error Handler.vi"("error in (no error)"=w940) -> ()  [unwired: 4 in, 5 out]
      }
      frame "CtrlRule: Remove" {
        n597 = Unbundle(w957) -> ("Group Rule out"=w959:T16)  [unwired: 1 out]
        n598 = in-place {
          in-place-border: w953 -> [w964]
          in-place-border: [w961] -> w952
          n599 = in-place-cluster #8(w959) -> ("Control Rules"=w963:T19[])
          n600 = Sort 1D Array(array=w964) -> (sorted array=w965:i32[])
          n601 = Reverse 1D Array(array=w965) -> (reversed array=w974:i32[])
          n602 = for {
            tunnel: w974 -> [w975] mode=indexing
            shift-right: [w977] -> w962
            shift-left: w963 -> [w976]
            n603 = Delete From Array(array=w976, index=w975) -> (array with subset deleted=w977:T19[])  [unwired: 1 in, 1 out]
          }
          n604 = Index Array(array=w965) -> (element=w973:i32)  [unwired: 1 in]
          n605 = Array Size(array=w962) -> (size(s)=w971:i32)
          n606 = Decrement(x=w971) -> (x-1=w966:i32)
          n607 = In Range and Coerce(upper limit=w966, x=w973, lower limit=0) -> (coerced(x)=w969:i32)  [unwired: 1 out]
          n608 = Less Than 0?(x=w966) -> (x < 0?=w970:bool)
          n609 = Build Array(w969) -> (w968:i32[])
          n610 = Select(t=i32[] [] ("CSS List"), s=w970, f=w968) -> (s? t:f=w961:i32[])
          n611 = in-place-cluster #8("Control Rules"=w962) -> (w958:T16)
        }
        n612 = local write "CtrlRule List"(w952) -> ()
        n613 = Bundle(cluster=w957, "Group Rule out"=w958) -> (w956:T28)  [unwired: 1 in]
        n614 = Concatenate Strings("Globals = Set;\n\nUpdate: Control Rules;\nCtrlRule: Update Controls = INIT;" ("string"), w960) -> (w955:string)
      }
      frame "CtrlRule: Dragged" {
        n615 = Unbundle(w981) -> ("Group Rule out"=w983:T16)  [unwired: 1 out]
        n616 = in-place {
          n617 = in-place-cluster #9(w983) -> ("Control Rules"=w986:T19[])
          n618 = property on="CtrlRule List" class="MCListbox (strict)"() -> ("ItemSyms"=w989:i32[])  [unwired: 2 in, 2 out]
          n619 = call "VIH Utility - UI - Drag and Drop Supporter (w Symbol Indices).vi"("Cmd"=enum16{"make symbols", "test D'n'D"}."test D'n'D", "Item Symbols"=w989) -> ("indices"=w987:i32[])  [unwired: 7 in, 2 out]
          n620 = for {
            tunnel: w987 -> [w992] mode=indexing
            tunnel: w986 -> [w991]
            tunnel: [w990] -> w985 mode=indexing
            n621 = Index Array(array=w991, index=w992) -> (element=w990:T19)
          }
          n622 = in-place-cluster #9("Control Rules"=w985) -> (w982:T16)
        }
        n623 = Concatenate Strings("Globals = Set;\n\nUpdate: Control Rules;\nCtrlRule: Update Controls = INIT;" ("string"), w984) -> (w979:string)
        n624 = Bundle(cluster=w981, "Group Rule out"=w982) -> (w980:T28)  [unwired: 1 in]
      }
      frame "CtrlRule: Apply" {
        n625 = Unbundle(w998) -> ("Group Rule out"=w1000:T16)  [unwired: 1 out]
        n626 = Decimal String To Number(string=w993, default (0L)=-1 ("default (0 I32)")) -> (number=w996:i32)  [unwired: 1 in, 1 out]
        n627 = in-place {
          in-place-border: w996 -> [w1005]
          n628 = in-place-cluster #10(w1000) -> ("Control Rules"=w1004:T19[])
          n629 = in-place {
            n630 = in-place-array #11(w1004, w1005) -> (w1019:T19)
            n631 = call <vilib>:"Trim Whitespace.vi"("string"="CtrlRule_CtrlID") -> ("trimmed string"=w1008:string)  [unwired: 1 in]
            n632 = call <vilib>:"Trim Whitespace.vi"("string"="CtrlRule_CustomName") -> ("trimmed string"=w1006:string)  [unwired: 1 in]
            n633 = Empty String/Path?(string/path=w1008) -> (empty?=w1012:bool)
            n634 = Select(t="<Control ID>", s=w1012, f=w1008) -> (s? t:f=w1010:string)
            n635 = Bundle By Name(cluster=w1019, "CtrlID"=w1010, "CustomRule"="CtrlRule_CustomRule", "DscrMode"="CtrlRule_DscrMode", "Description"="CtrlRule_Description", "ClusterMembers"="CtrlRule_ClustMembers", "EnumValues"="CtrlRule_EnumValues", "CustomName"=w1006) -> (w1018:T19)
            n636 = in-place-array #11(w1018) -> (w1003:T19[])  [unwired: 1 out]
          }
          n637 = in-place-cluster #10("Control Rules"=w1003) -> (w999:T16)
        }
        n638 = Concatenate Strings("Globals = Set;\n\nUpdate: Control Rules;\nCtrlRule: Update Controls;" ("string"), w1002) -> (w995:string)
        n639 = Bundle(cluster=w998, "Group Rule out"=w999) -> (w997:T28)  [unwired: 1 in]
      }
      frame "CtrlRule: Enable" {
        n640 = Unbundle(w1033) -> ("Group Rule out"=w1035:T16)  [unwired: 1 out]
        n641 = Match Pattern(string=w1020, regular expression="\\?") -> (before substring=w1024:string, after substring=w1026:string)  [unwired: 1 in, 2 out]
        n642 = Decimal String To Number(string=w1024) -> (number=w1027:i32)  [unwired: 2 in, 1 out]
        n643 = call "VIH Utility - STR - String to 1D Str Array.vi"("delimiter ('\\n')"="," ("delimiter ('\\n')"), "String in"=w1026) -> ("Array out"=w1028:string[])  [unwired: 5 in]
        n644 = Not Equal To 0?(x=w1027) -> (x != 0?=w1021:bool)
        n645 = Decimal String To Number(string=w1028, default (0L)=-1 ("default (0 I32)")) -> (number=w1022:i32[])  [unwired: 1 in, 1 out]
        n646 = in-place {
          in-place-border: w1022 -> [w1038]
          in-place-border: w1021 -> [w1037]
          n647 = in-place-cluster #12(w1035) -> ("Control Rules"=w1040:T19[])
          n648 = for {
            tunnel: w1038 -> [w1044] mode=indexing
            shift-right: [w1042] -> w1039
            shift-left: w1040 -> [w1043]
            tunnel: w1037 -> [w1041]
            n649 = in-place {
              in-place-border: w1041 -> [w1045]
              n650 = in-place-array #13(w1043, w1044) -> (w1047:T19)
              n651 = Bundle By Name(cluster=w1047, "CustomRule"=w1045) -> (w1046:T19)
              n652 = in-place-array #13(w1046) -> (w1042:T19[])  [unwired: 1 out]
            }
          }
          n653 = in-place-cluster #12("Control Rules"=w1039) -> (w1034:T16)
        }
        n654 = Concatenate Strings("Globals = Set;\n\nUpdate: Control Rules;\nCtrlRule: Update Controls;" ("string"), w1036) -> (w1031:string)
        n655 = Bundle(cluster=w1033, "Group Rule out"=w1034) -> (w1032:T28)  [unwired: 1 in]
      }
      frame "CtrlRule: Edit Enum Values" {
        n656 = Unbundle(w1054) -> ("Group Rule out"=w1056:T16)  [unwired: 1 out]
        n657 = Decimal String To Number(string=w1049, default (0L)=-1 ("default (0 I32)")) -> (number=w1052:i32)  [unwired: 1 in, 1 out]
        n658 = in-place {
          in-place-border: w1052 -> [w1062]
          in-place-border: w1048 -> [w1059]
          n659 = in-place-cluster #14(w1056) -> ("Control Rules"=w1061:T19[])
          n660 = in-place {
            in-place-border: w1059 -> [w1064]
            n661 = in-place-array #15(w1061, w1062) -> (w1068:T19)
            n662 = Unbundle By Name(w1068) -> ("EnumValDscr"=w1066:T20[], "CtrlID"=w1063:string)
            n663 = call "VIH Dialog - Enum Values.vi"("Control ID"=w1063, "EnumValDefs in"=w1066, "Project Tree"=w1064) -> ("OK out"=w1069:bool, "EnumValDefs out"=w1065:T20[])  [unwired: 7 in]
            n664 = case shown="True" w1069 {
              tunnel: [w1070 w1073] -> w1067
              tunnel: w1068 -> [w1070 w1072]
              tunnel: w1065 -> [_ w1071]
              frame False {
              }
              frame True {
                n665 = Bundle By Name(cluster=w1072, "EnumValDscr"=w1071) -> (w1073:T19)
              }
            }
            n666 = in-place-array #15(w1067) -> (w1060:T19[])  [unwired: 1 out]
          }
          n667 = in-place-cluster #14("Control Rules"=w1060) -> (w1055:T16)
        }
        n668 = Concatenate Strings("Globals = Set;\n\nUpdate: Control Rules;\nCtrlRule: Update Controls;" ("string"), w1058) -> (w1051:string)
        n669 = Bundle(cluster=w1054, "Group Rule out"=w1055) -> (w1053:T28)  [unwired: 1 in]
      }
      frame "------------------------------ 5" {
      }
      frame "CSS List: Update Controls" {
        n670 = Unbundle(w1081) -> ("Group Rule out"=w1080:T16)  [unwired: 1 out]
        n671 = Unbundle By Name(w1080) -> ("Source Paths.CSS Files"=w1079:path[])
        n672 = Index Array(array=w1078) -> (element=w1077:i32)  [unwired: 1 in]
        n673 = Empty Array?(array=w1078) -> (empty?=w1083:bool)
        n674 = call "VIH Utility - UI - Boolean to Control Disable Status.vi"("Status in"=w1083) -> ("Control Disable if True"=w1082:u8)  [unwired: 3 in, 1 out]
        n675 = Index Array(array=w1079, index=w1077) -> (element=→"CSS File":path)
        n676 = property on="%CSS List_Remove" class="Bool"("DisabledEnum"=w1082) -> ()  [unwired: 2 in, 2 out]
      }
      frame "CSS List: Make Selection Visible" {
        n677 = control-ref of="CSS List"() -> (w1091:refnum<vi>)
        n678 = property class="MCListbox (strict)"(reference=w1091) -> (reference out=w1090:refnum<vi>, "Value"=w1089:i32[])  [unwired: 1 in, 1 out]
        n679 = Empty Array?(array=w1089) -> (empty?=w1088:bool)
        n680 = Index Array(array=w1089) -> (element=w1087:i32)  [unwired: 1 in]
        n681 = Select(t=-1, s=w1088, f=w1087) -> (s? t:f=w1085:i32)
        n682 = call "VIH Utility - UI - Make Row Visible (MC Listbox).vi"("Row"=w1085, "MC Listbox Refnum"=w1090) -> ()  [unwired: 8 in, 2 out]
      }
      frame "CSS List: Add" {
        n683 = Array Size(array=w1097) -> (size(s)=w1095:i32)
        n684 = Unbundle(w1107) -> ("Group Rule out"=w1100:T16)  [unwired: 1 out]
        n685 = Array Max & Min(array=w1097) -> (max value=w1099:i32)  [unwired: 3 out]
        n686 = Unbundle By Name(w1100) -> ()  [unwired: 1 out]
        n687 = Less Or Equal To 0?(x=w1095) -> (x <= 0?=w1096:bool)
        n688 = Select(t=-1, s=w1096, f=w1099) -> (s? t:f=w1098:i32)
        n689 = call "File Dialog"("pattern (all files)"="*.css") -> ("selected paths"=w1103:path[], "error out"=w1104:errorcluster)  [unwired: 11 in, 2 out]
        n690 = case shown="No Error" w1104 {
          tunnel: w1100 -> [w1114 w1128]
          tunnel: [w1113 w1128] -> w1108
          tunnel: w1098 -> [w1112 _]
          tunnel: w1103 -> [w1111 _]
          tunnel: ["Globals = Set;\n\nUpdate: CSS List;\nCSS List: Make Selection Visible;\nCSS List: Update Controls;" ("string") _] -> w1101
          frame No Error {
            n691 = in-place {
              in-place-border: w1112 -> [w1120]
              in-place-border: w1111 -> [w1115]
              n692 = in-place-cluster #16(w1114) -> ("Source Paths.CSS Files"=w1121:path[])
              n693 = Increment(x=w1120) -> (x+1=w1119:i32)
              n694 = Array Size(array=w1121) -> (size(s)=w1122:i32)
              n695 = In Range and Coerce(upper limit=w1122, x=w1119, lower limit=0) -> (coerced(x)=w1118:i32)  [unwired: 1 out]
              n696 = Array Size(array=w1115) -> (size(s)=w1116:i32)
              n697 = for {
                N: w1116 -> [_]
                tunnel: w1118 -> [w1126]
                tunnel: [w1125] -> w1117 mode=indexing
                i -> [w1127]
                n698 = Add(x=w1126, y=w1127) -> (x+y=w1125:i32)
              }
              n699 = Insert Into Array(array=w1121, index=w1118, new element=w1115) -> (w1124:path[])
              n700 = in-place-cluster #16("Source Paths.CSS Files"=w1124) -> (w1113:T16)
              n701 = local write "CSS List"(w1117) -> ()
            }
          }
          frame Error {
          }
        }
        n702 = Concatenate Strings(w1101, w1109) -> (w1105:string)
        n703 = Bundle(cluster=w1107, "Group Rule out"=w1108) -> (w1106:T28)  [unwired: 1 in]
      }
      frame "CSS List: Remove" {
        n704 = Unbundle(w1133) -> ("Group Rule out"=w1135:T16)  [unwired: 1 out]
        n705 = in-place {
          in-place-border: w1129 -> [w1149]
          n706 = in-place-cluster #17(w1135) -> ("Source Paths.CSS Files"=w1150:path[])
          n707 = Sort 1D Array(array=w1149) -> (sorted array=w1139:i32[])
          n708 = Reverse 1D Array(array=w1139) -> (reversed array=w1148:i32[])
          n709 = for {
            tunnel: w1148 -> [w1151] mode=indexing
            shift-right: [w1153] -> w1138
            shift-left: w1150 -> [w1152]
            n710 = Delete From Array(array=w1152, index=w1151) -> (array with subset deleted=w1153:path[])  [unwired: 1 in, 1 out]
          }
          n711 = Index Array(array=w1139) -> (element=w1147:i32)  [unwired: 1 in]
          n712 = Array Size(array=w1138) -> (size(s)=w1145:i32)
          n713 = Decrement(x=w1145) -> (x-1=w1140:i32)
          n714 = In Range and Coerce(upper limit=w1140, x=w1147, lower limit=0) -> (coerced(x)=w1143:i32)  [unwired: 1 out]
          n715 = Less Than 0?(x=w1140) -> (x < 0?=w1144:bool)
          n716 = Build Array(w1143) -> (w1142:i32[])
          n717 = in-place-cluster #17("Source Paths.CSS Files"=w1138) -> (w1134:T16)
          n718 = Select(t=i32[] [] ("CSS List"), s=w1144, f=w1142) -> (s? t:f=w1137:i32[])
          n719 = local write "CSS List"(w1137) -> ()
        }
        n720 = Concatenate Strings("Globals = Set;\n\nUpdate: CSS List;\nCSS List: Make Selection Visible;\nCSS List: Update Controls;" ("string"), w1136) -> (w1131:string)
        n721 = Bundle(cluster=w1133, "Group Rule out"=w1134) -> (w1132:T28)  [unwired: 1 in]
      }
      frame "CSS List: Dragged" {
        n722 = Unbundle(w1157) -> ("Group Rule out"=w1159:T16)  [unwired: 1 out]
        n723 = in-place {
          n724 = in-place-cluster #18(w1159) -> ("Source Paths.CSS Files"=w1162:path[])
          n725 = property on="CSS List" class="MCListbox (strict)"() -> ("ItemSyms"=w1165:i32[])  [unwired: 2 in, 2 out]
          n726 = call "VIH Utility - UI - Drag and Drop Supporter (w Symbol Indices).vi"("Cmd"=enum16{"make symbols", "test D'n'D"}."test D'n'D", "Item Symbols"=w1165) -> ("indices"=w1163:i32[])  [unwired: 7 in, 2 out]
          n727 = for {
            tunnel: w1163 -> [w1168] mode=indexing
            tunnel: w1162 -> [w1167]
            tunnel: [w1166] -> w1161 mode=indexing
            n728 = Index Array(array=w1167, index=w1168) -> (element=w1166:path)
          }
          n729 = in-place-cluster #18("Source Paths.CSS Files"=w1161) -> (w1158:T16)
        }
        n730 = Concatenate Strings("Globals = Set;\n\nUpdate: CSS List;\n\nCSS List: Update Controls;" ("string"), w1160) -> (w1155:string)
        n731 = Bundle(cluster=w1157, "Group Rule out"=w1158) -> (w1156:T28)  [unwired: 1 in]
      }
      frame "------------------------------ 6" {
      }
      frame "JS List: Update Controls" {
        n732 = Unbundle(w1176) -> ("Group Rule out"=w1175:T16)  [unwired: 1 out]
        n733 = Unbundle By Name(w1175) -> ("Source Paths.JS Files"=w1174:path[])
        n734 = Index Array(array=w1171) -> (element=w1173:i32)  [unwired: 1 in]
        n735 = Empty Array?(array=w1171) -> (empty?=w1178:bool)
        n736 = call "VIH Utility - UI - Boolean to Control Disable Status.vi"("Status in"=w1178) -> ("Control Disable if True"=w1177:u8)  [unwired: 3 in, 1 out]
        n737 = Index Array(array=w1174, index=w1173) -> (element=→"JS File":path)
        n738 = property on="%JS List_Remove" class="Bool"("DisabledEnum"=w1177) -> ()  [unwired: 2 in, 2 out]
      }
      frame "JS List: Make Selection Visible" {
        n739 = control-ref of="JS List"() -> (w1186:refnum<vi>)
        n740 = property class="MCListbox (strict)"(reference=w1186) -> (reference out=w1185:refnum<vi>, "Value"=w1184:i32[])  [unwired: 1 in, 1 out]
        n741 = Empty Array?(array=w1184) -> (empty?=w1183:bool)
        n742 = Index Array(array=w1184) -> (element=w1182:i32)  [unwired: 1 in]
        n743 = Select(t=-1, s=w1183, f=w1182) -> (s? t:f=w1180:i32)
        n744 = call "VIH Utility - UI - Make Row Visible (MC Listbox).vi"("Row"=w1180, "MC Listbox Refnum"=w1185) -> ()  [unwired: 8 in, 2 out]
      }
      frame "JS List: Add" {
        n745 = Array Size(array=w1190) -> (size(s)=w1192:i32)
        n746 = Unbundle(w1202) -> ("Group Rule out"=w1195:T16)  [unwired: 1 out]
        n747 = Unbundle By Name(w1195) -> ()  [unwired: 1 out]
        n748 = Array Max & Min(array=w1190) -> (max value=w1194:i32)  [unwired: 3 out]
        n749 = Less Or Equal To 0?(x=w1192) -> (x <= 0?=w1193:bool)
        n750 = Select(t=-1, s=w1193, f=w1194) -> (s? t:f=w1191:i32)
        n751 = call "File Dialog2"("pattern (all files)"="*.js") -> ("selected paths"=w1198:path[], "error out"=w1199:errorcluster)  [unwired: 11 in, 2 out]
        n752 = case shown="No Error" w1199 {
          tunnel: w1195 -> [w1209 w1223]
          tunnel: [w1208 w1223] -> w1203
          tunnel: w1191 -> [w1207 _]
          tunnel: w1198 -> [w1206 _]
          tunnel: ["Globals = Set;\n\nUpdate: JS List;\nJS List: Make Selection Visible;\nJS List: Update Controls;" ("string") _] -> w1196
          frame No Error {
            n753 = in-place {
              in-place-border: w1207 -> [w1215]
              in-place-border: w1206 -> [w1210]
              n754 = in-place-cluster #19(w1209) -> ("Source Paths.JS Files"=w1216:path[])
              n755 = Increment(x=w1215) -> (x+1=w1214:i32)
              n756 = Array Size(array=w1216) -> (size(s)=w1217:i32)
              n757 = In Range and Coerce(upper limit=w1217, x=w1214, lower limit=0) -> (coerced(x)=w1213:i32)  [unwired: 1 out]
              n758 = Array Size(array=w1210) -> (size(s)=w1211:i32)
              n759 = for {
                N: w1211 -> [_]
                tunnel: w1213 -> [w1221]
                tunnel: [w1220] -> w1212 mode=indexing
                i -> [w1222]
                n760 = Add(x=w1221, y=w1222) -> (x+y=w1220:i32)
              }
              n761 = Insert Into Array(array=w1216, index=w1213, new element=w1210) -> (w1219:path[])
              n762 = in-place-cluster #19("Source Paths.JS Files"=w1219) -> (w1208:T16)
              n763 = local write "JS List"(w1212) -> ()
            }
          }
          frame Error {
          }
        }
        n764 = Concatenate Strings(w1196, w1204) -> (w1200:string)
        n765 = Bundle(cluster=w1202, "Group Rule out"=w1203) -> (w1201:T28)  [unwired: 1 in]
      }
      frame "JS List: Remove" {
        n766 = Unbundle(w1228) -> ("Group Rule out"=w1230:T16)  [unwired: 1 out]
        n767 = in-place {
          in-place-border: w1224 -> [w1244]
          n768 = in-place-cluster #20(w1230) -> ("Source Paths.JS Files"=w1245:path[])
          n769 = Sort 1D Array(array=w1244) -> (sorted array=w1242:i32[])
          n770 = Reverse 1D Array(array=w1242) -> (reversed array=w1243:i32[])
          n771 = for {
            tunnel: w1243 -> [w1246] mode=indexing
            shift-right: [w1248] -> w1239
            shift-left: w1245 -> [w1247]
            n772 = Delete From Array(array=w1247, index=w1246) -> (array with subset deleted=w1248:path[])  [unwired: 1 in, 1 out]
          }
          n773 = Index Array(array=w1242) -> (element=w1241:i32)  [unwired: 1 in]
          n774 = Array Size(array=w1239) -> (size(s)=w1238:i32)
          n775 = Decrement(x=w1238) -> (x-1=w1232:i32)
          n776 = In Range and Coerce(upper limit=w1232, x=w1241, lower limit=0) -> (coerced(x)=w1236:i32)  [unwired: 1 out]
          n777 = Less Than 0?(x=w1232) -> (x < 0?=w1237:bool)
          n778 = Build Array(w1236) -> (w1235:i32[])
          n779 = Select(t=i32[] [] ("CSS List"), s=w1237, f=w1235) -> (s? t:f=w1233:i32[])
          n780 = in-place-cluster #20("Source Paths.JS Files"=w1239) -> (w1229:T16)
          n781 = local write "JS List"(w1233) -> ()
        }
        n782 = Concatenate Strings("Globals = Set;\n\nUpdate: JS List;\nJS List: Make Selection Visible;\nJS List: Update Controls;" ("string"), w1231) -> (w1226:string)
        n783 = Bundle(cluster=w1228, "Group Rule out"=w1229) -> (w1227:T28)  [unwired: 1 in]
      }
      frame "JS List: Dragged" {
        n784 = Unbundle(w1252) -> ("Group Rule out"=w1254:T16)  [unwired: 1 out]
        n785 = in-place {
          n786 = in-place-cluster #21(w1254) -> ("Source Paths.JS Files"=w1257:path[])
          n787 = property on="JS List" class="MCListbox (strict)"() -> ("ItemSyms"=w1260:i32[])  [unwired: 2 in, 2 out]
          n788 = call "VIH Utility - UI - Drag and Drop Supporter (w Symbol Indices).vi"("Cmd"=enum16{"make symbols", "test D'n'D"}."test D'n'D", "Item Symbols"=w1260) -> ("indices"=w1258:i32[])  [unwired: 7 in, 2 out]
          n789 = for {
            tunnel: w1258 -> [w1263] mode=indexing
            tunnel: w1257 -> [w1262]
            tunnel: [w1261] -> w1256 mode=indexing
            n790 = Index Array(array=w1262, index=w1263) -> (element=w1261:path)
          }
          n791 = in-place-cluster #21("Source Paths.JS Files"=w1256) -> (w1253:T16)
        }
        n792 = Concatenate Strings("Globals = Set;\n\nUpdate: JS List;\n\nJS List: Update Controls;" ("string"), w1255) -> (w1250:string)
        n793 = Bundle(cluster=w1252, "Group Rule out"=w1253) -> (w1251:T28)  [unwired: 1 in]
      }
      frame "------------------------------ 7" {
      }
      frame "Control Appearance" {
        (unwired) "Control"
      }
    }
  }
  n794 = while {
    shift-right: [w1272] -> _
    shift-left: "INIT;" -> [w1275]
    tunnel: w2 -> [w1269]
    tunnel: w3 -> [w1268]
    stop <- w1270 stop-if-true
    n795 = call "VIH Utility - APP - State Queue Parser (STR).vi"("input queue"=w1275) -> ("state"=w1274:string, "remained queue"=w1271:string, "complete state specifier"=w1273:string)  [unwired: 5 in, 1 out]
    n796 = case shown="\"\"" w1274 {
      tunnel: w1273 -> [w1281 _ _ _]
      tunnel: [w1276 w1286 w1288 w1296] -> w1272
      tunnel: w1271 -> [w1277 w1286 w1288 w1295]
      tunnel: [_ _ TRUE _] -> w1270
      tunnel: w1269 -> [_ _ w1287 w1299]
      tunnel: w1268 -> [_ _ _ w1294]
      frame Default {
        n797 = property class="VI"() -> ("Name"=w1280:string)  [unwired: 2 in, 2 out]
        n798 = Format Into String(format string="%s\n(Communication Loop)\n\nUnknown state specifier:\n%s", w1280, w1281) -> (resulting string=w1284:string)  [unwired: 2 in, 1 out]
        n799 = Two Button Dialog(message=w1284, 1:"HALT" ("F button name (\"Cancel\")"), 2:"Continue" ("T button name (\"OK\")")) -> (T button?=w1278:bool)
        n800 = Select(t=w1277, s=w1278, f="HALT;") -> (s? t:f=w1276:string)
      }
      frame "INIT" {
      }
      frame "HALT" {
        n801 = Release Queue(queue=w1287) -> ()  [unwired: 2 in, 3 out]
      }
      frame "" {
        n802 = Dequeue Element(queue=w1299, timeout in ms (-1)=200) -> (element=w1290:T8, error out=w1298:errorcluster)  [unwired: 1 in, 2 out]
        n803 = Unbundle By Name(w1290) -> ("Action"=w1292:string)
        n804 = Empty String/Path?(string/path=w1292) -> (empty?=w1291:bool)
        n805 = case shown="False" w1291 {
          tunnel: w1294 -> [w1301 _]
          tunnel: w1290 -> [w1300 _]
          frame False {
            n806 = Generate User Event(user event=w1301, event data cluster=w1300) -> ()  [unwired: 2 in, 2 out]
          }
          frame True {
          }
        }
        n807 = Select(t="HALT;", s=w1298, f=w1295) -> (s? t:f=w1296:string)
      }
    }
  }
